vi "ACE401.vi"() -> ()   [LabVIEW 2018]
uses:
  <vilib>/registry/registry.llb/Registry RtKey.ctl
  <vilib>/registry/registry.llb/Registry SAM.ctl
  <vilib>/Utility/miscctls.llb/LVRowAndColumnUnsignedTypeDef.ctl
  <vilib>/Utility/cursorutil.llb/Set Cursor (Icon Pict).vi
  <vilib>/registry/registry.llb/Read Registry Value Simple STR.vi
panel:
  in  "Firebase URL":string
  in  "Enable IoT":bool
  out "Exp":string
  out "current time":timestamp format="%<%d/%m/%Y - %I:%M:%S %p>T"
  in  "Radio Buttons":T1(radio)
  out "Flag":bool
  in  "Action":bool
  in  "Stop Flag":bool
  out "Tank":dbl(slide) scale=0.0..100.0 scale format="%#.1g"
  in  "OP_1 2":dbl=50.0 caption="SP %" format="%3.1f"
  in  "SP_1":dbl=50.0 caption="SP %" format="%3.1f"
  in  "PV_1":dbl caption="PV %" format="%3.1f"
  out "Boolean 3":bool
  out "Multi-Segment Pipe 5":bool(c317)
  out "Multi-Segment Pipe 4":bool(c317)
  out "Multi-Segment Pipe 3":bool(c317)
  out "Multi-Segment Pipe 2":bool(c317)
  out "Boolean":bool
  out "Tank 2":dbl(slide)=58.333333333333336 scale=0.0..100.0
  out "Multi-Segment Pipe":bool(c317)
  out "Boolean 2":bool
  out "Enum":T2(ring)
  in  "Experiment Selection":u16(ring)=5 items=["On / Off Control", "P Mode", "PI Mode", "PD Mode", "PID Mode"]
  in  "Tab Control 3":enum32{"Plot2"}(tab)
  out "Waveform Chart":T3(graph)={"Register Value"=20.0, "Value"=0.0, "Register Value"=0.0}
  in  "Run":bool caption="Blank Button"
  out "Log":bool
  in  "Log Button":bool caption="Blank Button"
  in  "Constant PV":bool
  in  "Constant Outflow":bool
  in  "Anti Reset Windup":bool=TRUE
  in  "Bumpless Transfer":bool=TRUE
  in  "Pause":bool caption="Blank Button"
  in  "Single Step":bool caption="Blank Button"
  in  "Stop":bool caption="Blank Button"
  in  "Save Log":bool caption="Blank Button"
  in  "Clear":bool caption="Blank Button"
  in  "Export":bool caption="Blank Button"
  in  "help":bool caption="Blank Button"
  in  "Home":bool caption="Blank Button"
  in  "Tab Control 2":T4(tab)
  in  "Steady State Flow \n@50% of PV(LPH)":dbl(slide)=40.0 min=0.0 step=1.0 scale=0.0..100.0
  in  "Time Lag (s)":u32(slide)=1 min=1 max=10 step=1 scale=0.0..10.0
  in  "Max. Inflow (LPH)":dbl(slide)=100.0 min=0.0 step=1.0 scale=0.0..400.0
  in  "Tank Height  (cms)":dbl(slide)=25.0 min=10.0 step=1.0 scale=0.0..200.0
  in  "Tank Diameter  (cms)":dbl(slide)=10.0 min=5.0 step=1.0 scale=0.0..40.0
  in  "A / M":bool
  in  "Set Point (%)":dbl(slide)=50.0 min=0.0 max=100.0 step=0.1 scale=0.0..100.0
  in  "Process Variable (%)":dbl(slide) min=0.0 max=100.0 step=1.0 scale=0.0..100.0
  in  "Controller Output (%)":dbl(slide)=100.0 min=0.0 max=100.0 step=0.1 scale=0.0..100.0
  in  "DT s":dbl(slide)=1.0 caption="Derivative Time (s)" min=0.0 max=100.0 step=0.1 scale=0.0..20.0
  in  "IT s":dbl(slide)=30.0 caption="Integral Time (s)" min=0.0 max=100.0 step=0.1 scale=0.0..1000.0
  in  "PB %":dbl(slide)=20.0 caption="Proportional Band (%)" min=0.0 max=100.0 step=0.1 scale=0.0..400.0
  in  "Bias (%)":dbl(slide)=40.0 min=0.0 max=100.0 step=0.1 scale=0.0..100.0
  in  "Hystresis (%)":dbl(slide)=2.0 min=0.0 max=100.0 step=0.1 scale=0.0..20.0
  in  "Out Flow (%)":dbl(slide)=40.0 min=0.0 max=100.0 step=0.1 scale=0.0..100.0
  in  "Add Load":bool
  in  "PB Contribution (%)":dbl=60.0 min=0.0 max=100.0 step=0.1 format="%#.1f"
  in  "IOP":dbl=1.0 caption="IT Contribution (%)" min=0.0 max=100.0 step=0.1 format="%#.2f"
  in  "DOP":dbl=1.0 caption="DT Contribution (%)" min=0.0 max=100.0 step=0.1 format="%#.2f"
  in  "Load":dbl(slide)=10.0 caption="Load (%)" min=-50.0 max=50.0 step=1.0 scale=-100.0..100.0
  out "Table":string[][](table)
  out "out1":dbl=2.0
  in  "Array":dbl[](array[numeric])=[0.0, 0.0, 0.0, 0.0, 0.0, 0.0, 0.0, 0.0, 0.0, 0.0]
  out "err":dbl
  out "dh":dbl=2.0
  out "K":dbl
  out "Area":dbl
  out "qi":dbl=100.0
  out "i2":dbl
  out "Log Count":dbl
  out "PV % 2":dbl caption="PV %" format="%#.1f"
  out "SP % 2":dbl caption="SP %" format="%#.1f"
  # "Advanced Control Equipments\n(Ahead Traditional Control)"
  # "Two Position & PID Simulator (ACE 401)"
  # "Study Parameters"
  # "I / P Converter"
  # "Level Controller"
  # "Rotameter"
  # "Process Tank"
  # "Control Valve"
  # "Manual\nDrain Valve"
  # "Level Transmitter"
  # "Supply Tank"
  # "Pump"
  # "Select Experiment"
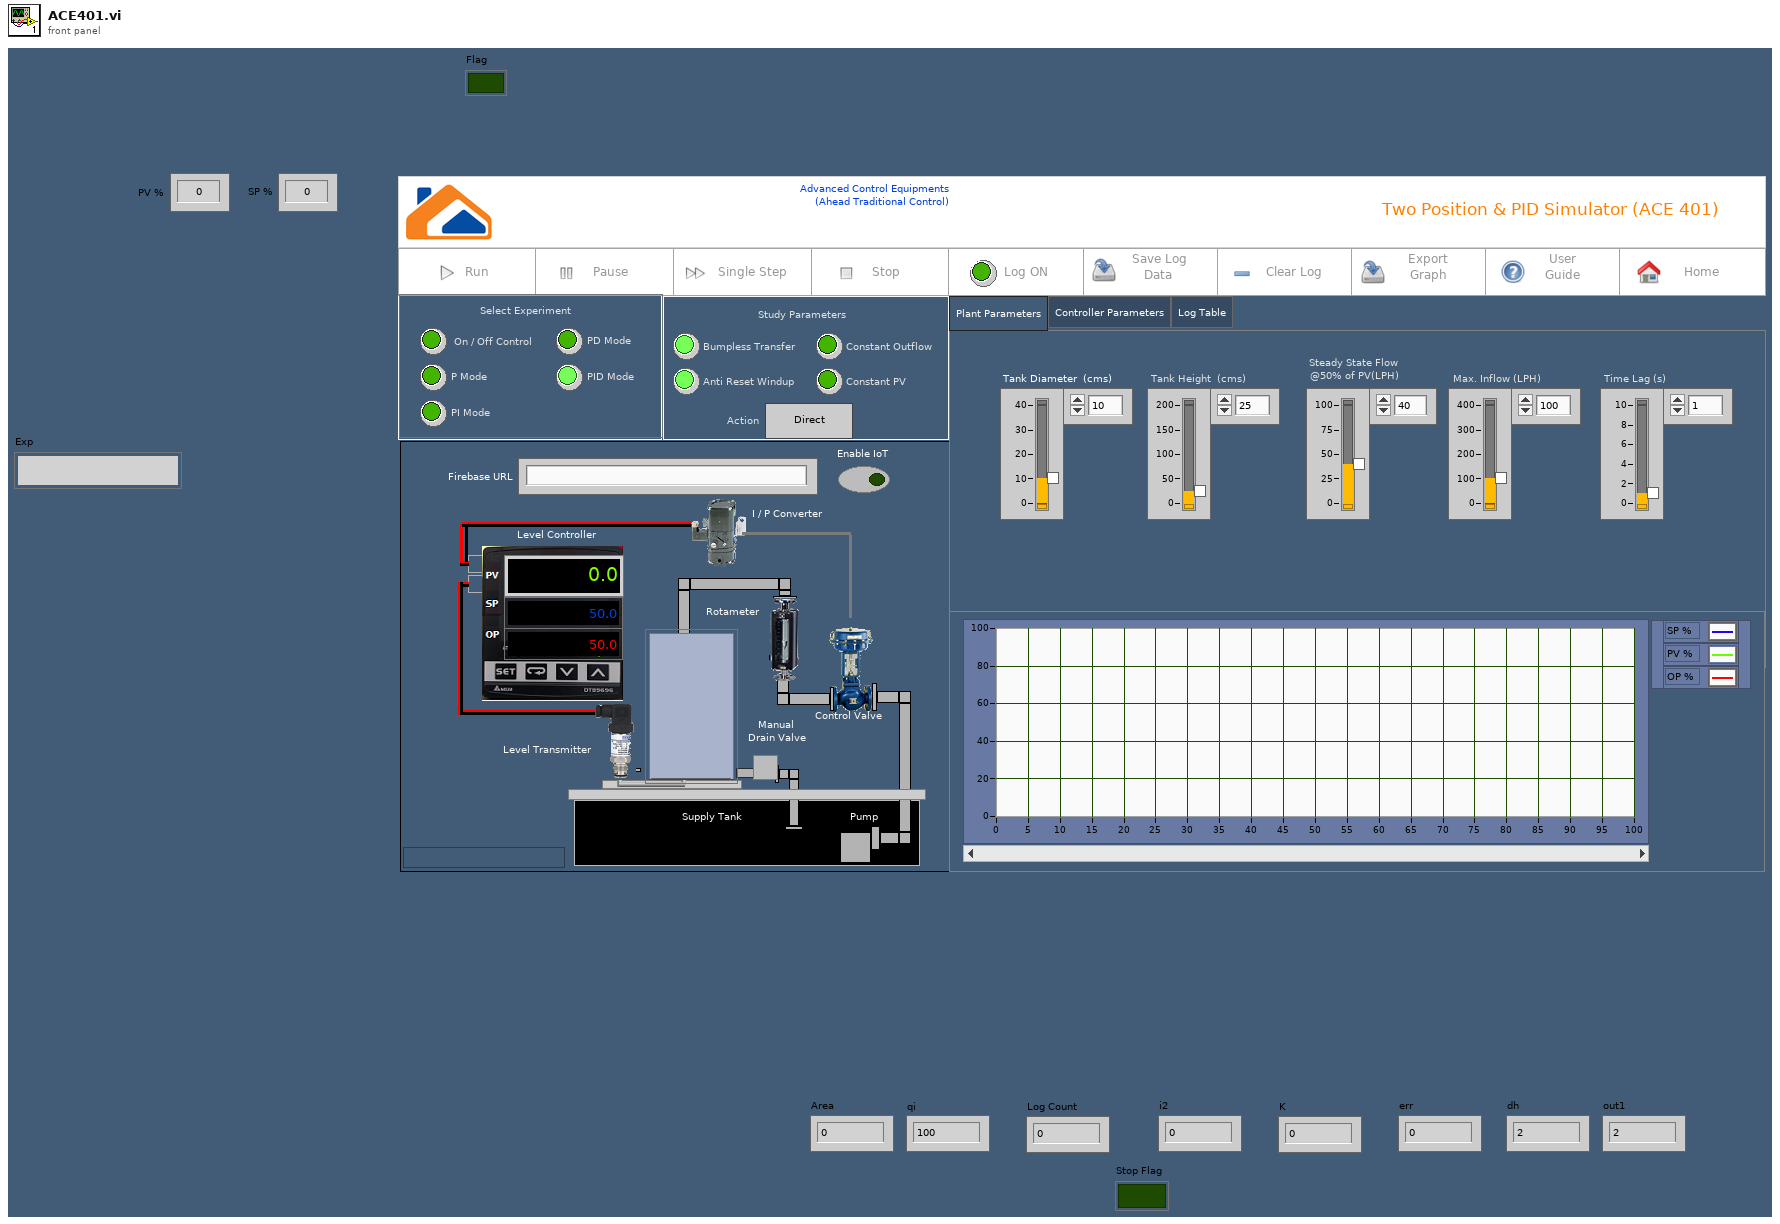
[diagram p1: front panel]
types:
  T1 = enum32{"PID Mode", "On / Off Control", "P Mode", "PI Mode", "PD Mode"}
  T2 = enum16{"Initialize", "Select Exp", "Play", "Stop", "Error", "Pause", "MainPage", "Wait"}
  T3 = cluster{"Register Value":dbl, "Value":dbl, "Register Value":dbl}
  T4 = enum32{"Plant Parameters", "Controller Parameters", "Log Table"}
  T5 = enum16{"Initialize", "Select Exp", "Play", "Stop", "Error", "Pause", "MainPage"}
  T6 = enum32{"Page Enabled", "Page Disabled", "Page Disabled & Grayed"}
  T7 = cluster{"Register Value":dbl, "Value":dbl, "Register Value":dbl}[]
  T8 = typedef "LVRowAndColumnUnsignedTypeDef.ctl" = cluster{"Row":u32, "Column":u32}
  T9 = enum8{"Enabled", "Disabled", "Disabled and Grayed Out"}
  T10 = cluster{"Set Point (%)":dbl, "pv1":dbl, "upper limit":dbl}
  T11 = typedef "Registry SAM.ctl" = enum32{"KEY_QUERY_VALUE", "KEY_SET_VALUE", "KEY_CREATE_SUB_KEY", "KEY_ENUMERATE_SUB_KEYS", "KEY_NOTIFY", "KEY_CREATE_LINK", "KEY_READ", "KEY_WRITE", "KEY_ALL_ACCESS", "KEY_READ | KEY_WRITE"}
  T12 = typedef "Registry RtKey.ctl" = enum32{"HKEY_CLASSES_ROOT", "HKEY_CURRENT_USER", "HKEY_LOCAL_MACHINE", "HKEY_USERS", "HKEY_PERFORMANCE_DATA", "HKEY_CURRENT_CONFIG", "HKEY_DYN_DATA"}
  T13 = typedef "imagedata.ctl" = cluster{"image type":i32, "image depth":i32, "image":u8[], "mask":u8[], "colors":u32[], "Rectangle":cluster{"left":i16, "top":i16, "right":i16, "bottom":i16}}
  T14 = typedef "Registry refnum.ctl" = refnum<k1>
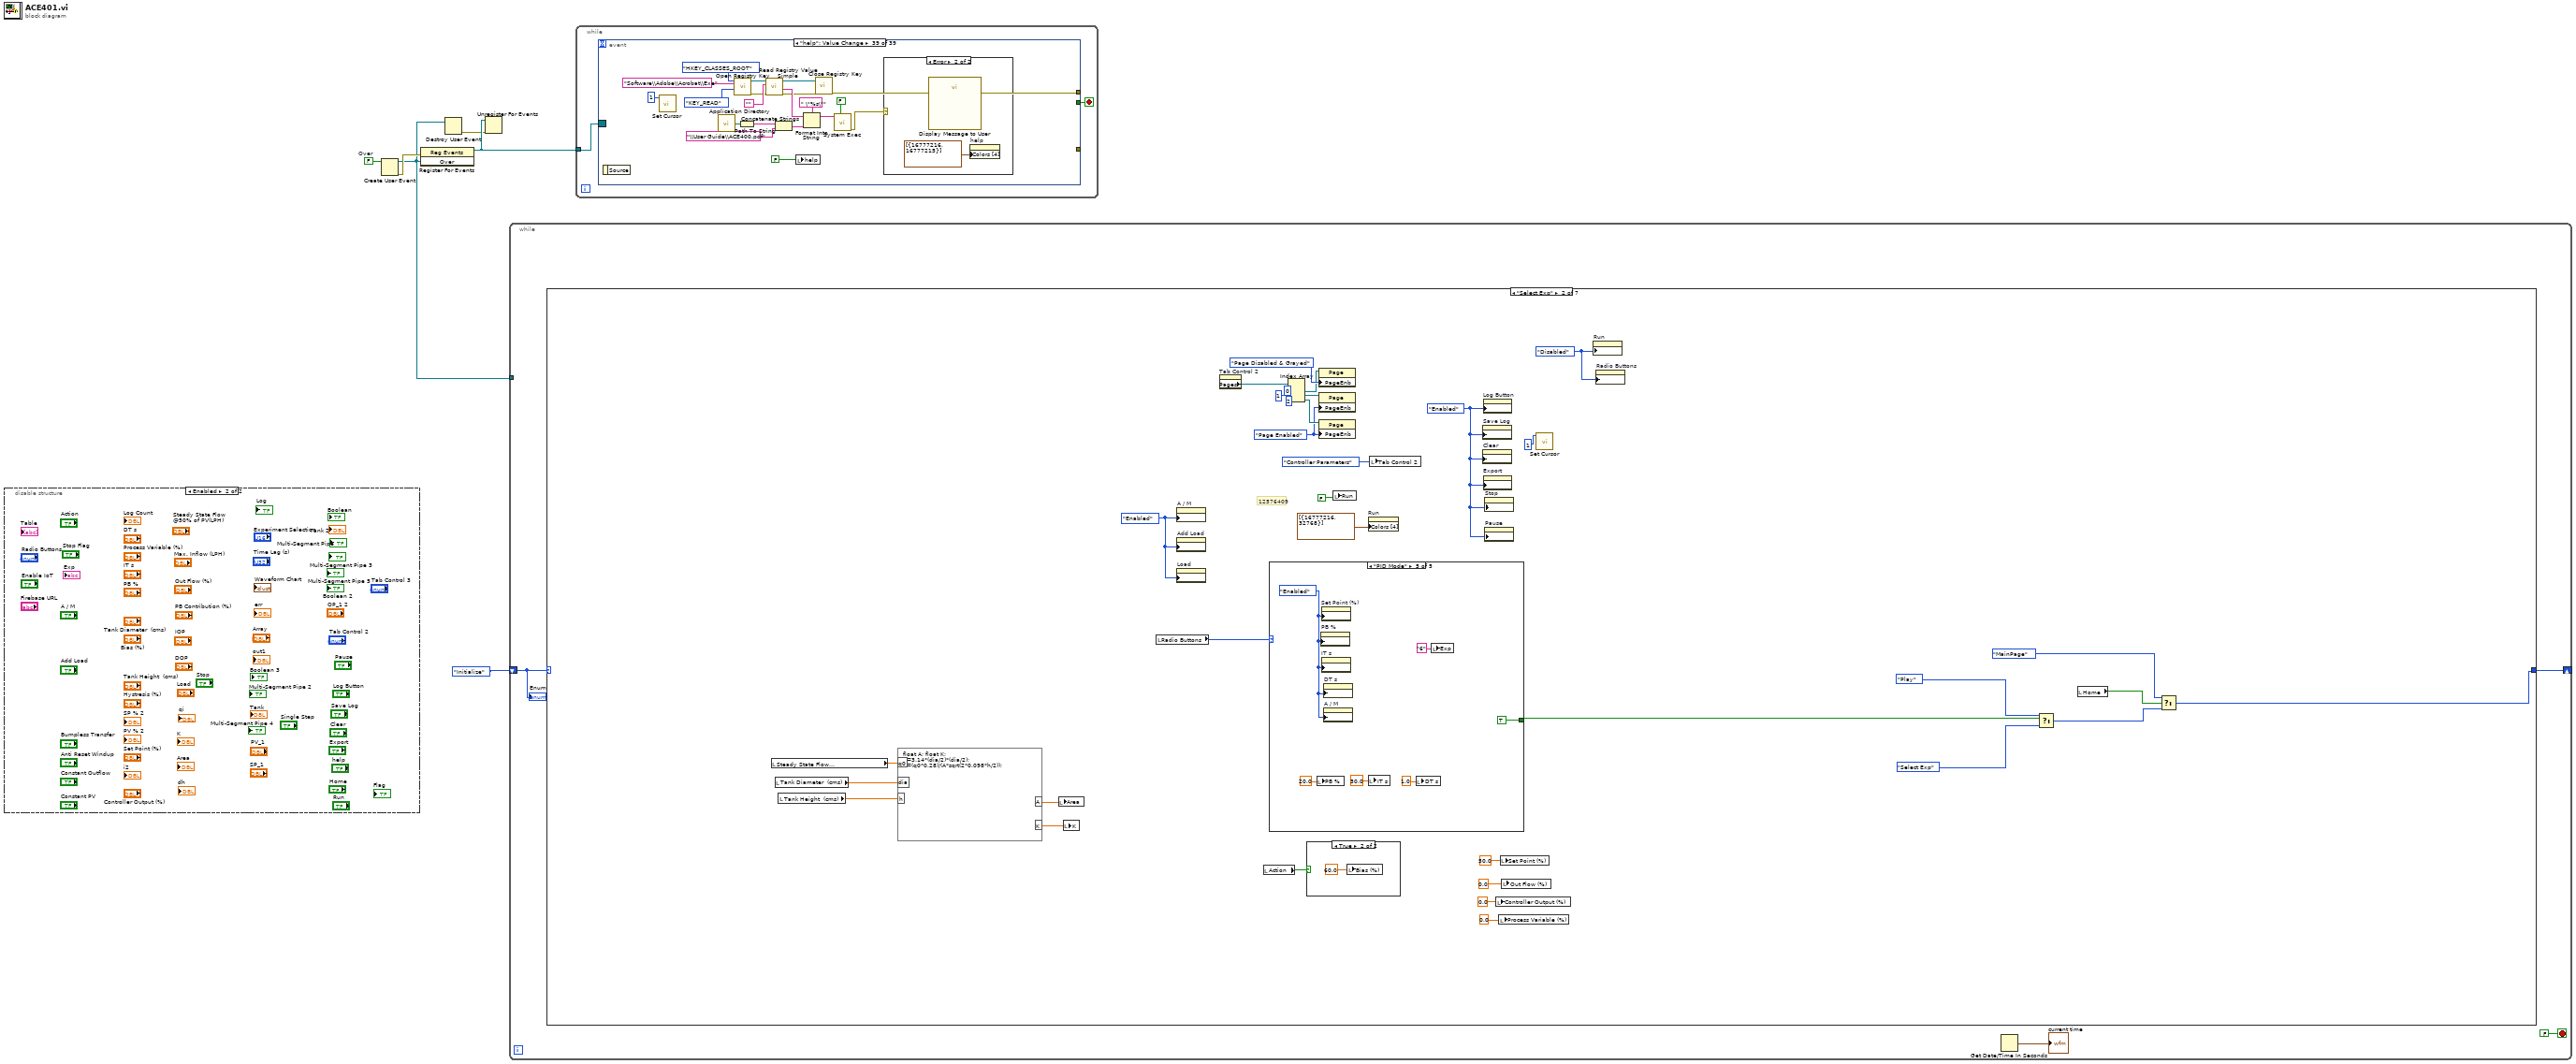
[diagram p0: block diagram]
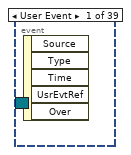
[diagram p2: hidden frame]
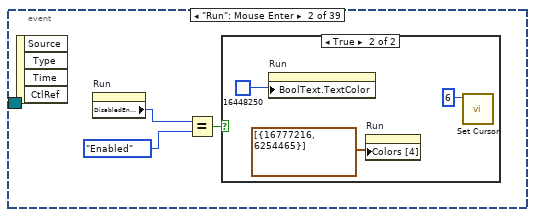
[diagram p3: hidden frame]
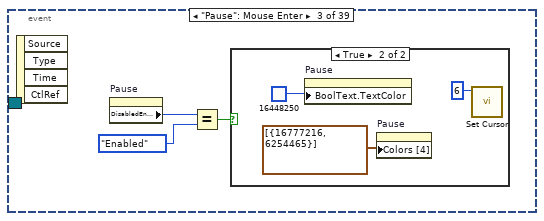
[diagram p5: hidden frame]
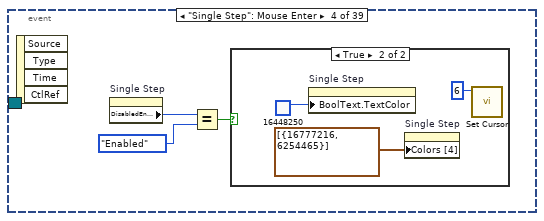
[diagram p7: hidden frame]
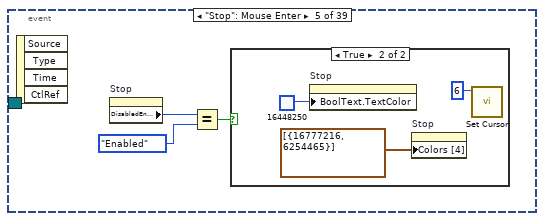
[diagram p9: hidden frame]
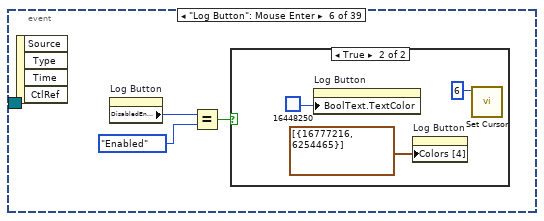
[diagram p11: hidden frame]
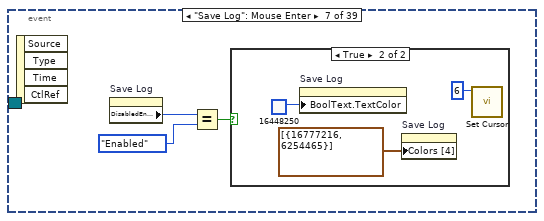
[diagram p13: hidden frame]
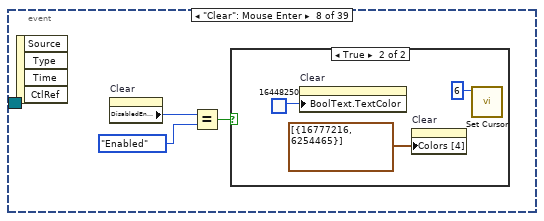
[diagram p15: hidden frame]
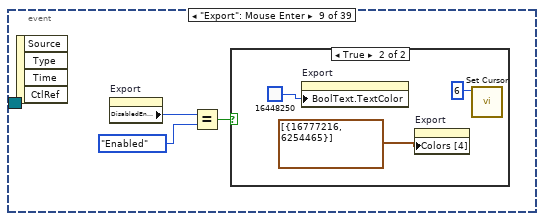
[diagram p17: hidden frame]
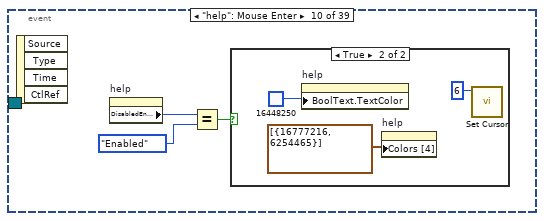
[diagram p19: hidden frame]
diagram:
  w4 = FALSE  # Over
  n1 = disable-structure shown="Enabled" {
    frame Disabled {
    }
    frame Enabled {
    }
  }
  n2 = Create User Event(user event datatype=w4) -> (user event=w2:refnum<user-event>, error out=w5:errorcluster)  [unwired: 1 in]
  n3 = register-events(error in=w5, w2) -> (reference out=w3:refnum<event-registration>)  [unwired: 1 in, 1 out]
  n4 = Unregister For Events(event registration refnum=w3) -> (error out=w1:errorcluster)  [unwired: 1 in]
  n5 = Destroy User Event(user event=w2, error in=w1) -> ()  [unwired: 1 out]
  n6 = while {
    shift-right: [w10] -> _
    shift-left: T2."Initialize" -> [w8]
    tunnel: w2 -> [_]
    stop <- FALSE stop-if-true
    n7 = case shown="\"Select Exp\"" w8 {
      tunnel: [w17 w75 w125 w682 w692 w698 _] -> w10
      frame "Initialize", Default {
        n8 = flat-sequence {
          frame #0 {
            w19 = T9."Disabled and Grayed Out" ("Disabled")
            w18 = T9."Enabled" ("Disabled")
            w22 = FALSE ("Stop Button")
            w31 = T6."Page Disabled & Grayed" ("Page Enabled State")
            w20 = T9."Disabled" ("Disabled")
            w21 = FALSE ("Log Button")
            w37 = 0.0 ("Log Count")
            n9 = local read "Action"() -> (w23:bool)
            n10 = property on="A / M" class="Bool (strict)"("BoolText.Text"="Auto" ("Boolean Text.Text")) -> ()  [unwired: 2 in, 2 out]
            n11 = case shown="False" w23 {
              frame True {
                n12 = property on="Array" class="Arr (strict)"("Value"=dbl[] [100.0, 100.0, 100.0, 100.0, 100.0, 100.0, 100.0, 100.0, 100.0, 100.0] ("Array")) -> ()  [unwired: 2 in, 2 out]
              }
              frame False {
                n13 = property on="Array" class="Arr (strict)"("Value"=dbl[] [0.0, 0.0, 0.0, 0.0, 0.0, 0.0, 0.0, 0.0, 0.0, 0.0] ("Array")) -> ()  [unwired: 2 in, 2 out]
              }
            }
            n14 = invoke on="Table" class="Tbl (strict)" method="Reinit To Default"() -> ()  [unwired: 3 in, 3 out]
            n15 = property on="Table" class="Tbl (strict)"("Value"=string[][] [] ("Table")) -> ()  [unwired: 2 in, 2 out]
            n16 = local write "Log Button"(w21) -> ()
            n17 = local write "Single Step"(w21) -> ()
            n18 = local write "Stop Flag"(w21) -> ()
            n19 = local write "A / M"(w21) -> ()
            n20 = local write "Pause"(w21) -> ()
            n21 = local write "Clear"(w21) -> ()
            n22 = local write "Stop"(w21) -> ()
            n23 = property on="Waveform Chart" class="WFChart (strict)"("History Data"=T7 []) -> ()  [unwired: 2 in, 2 out]
            n24 = local write "Single Step"(w22) -> ()
            n25 = local write "Pause"(w22) -> ()
            n26 = local write "Stop"(w22) -> ()
            n27 = local write "Process Variable (%)"(w37) -> ()
            n28 = local write "PB Contribution (%)"(w37) -> ()
            n29 = property on="Tab Control 2" class="TabCtl (strict)"() -> ("Pages"=w28:refnum<vi>[])  [unwired: 2 in, 2 out]
            n30 = local write "Log Count"(w37) -> ()
            n31 = local write "Bias (%)"(w37) -> ()
            n32 = local write "OP_1 2"(w37) -> ()
            n33 = local write "i2"(w37) -> ()
            n34 = local write "DOP"(w37) -> ()
            n35 = local write "PV_1"(w37) -> ()
            n36 = local write "IOP"(w37) -> ()
            n37 = local write "dh"(w37) -> ()
            n38 = Index Array(array=w28, index #1=0 ("index"), index #2=1 ("index"), index #3=2 ("index")) -> (element #1=w25:refnum<vi>, element #2=w30:refnum<vi>, element #3=w32:refnum<vi>)
            n39 = local write "qi"(100.0 ("qi")) -> ()
            n40 = local write "Tab Control 2"(T4."Plant Parameters" ("Tab Control 2")) -> ()
            n41 = local write "SP_1"(50.0 ("qi")) -> ()
            n42 = property on="Table" class="Tbl (strict)"("Index Values"=T8 {"Row"=0, "Column"=0}) -> ()  [unwired: 2 in, 2 out]
            n43 = property on="Log" class="Bool (strict)"("Blinking"=FALSE) -> ()  [unwired: 2 in, 2 out]
            n44 = property class="Page"(reference=w25, "PageEnb"=T6."Page Enabled" ("Page Enabled State")) -> ()  [unwired: 1 in, 2 out]
            n45 = property class="Page"(reference=w30, "PageEnb"=w31) -> ()  [unwired: 1 in, 2 out]
            n46 = property class="Page"(reference=w32, "PageEnb"=w31) -> ()  [unwired: 1 in, 2 out]
            n47 = property on="Log Button" class="Bool (strict)"("DisabledEnum"=w20) -> ()  [unwired: 2 in, 2 out]
            n48 = property on="Save Log" class="Bool (strict)"("DisabledEnum"=w20) -> ()  [unwired: 2 in, 2 out]
            n49 = property on="Clear" class="Bool (strict)"("DisabledEnum"=w20) -> ()  [unwired: 2 in, 2 out]
            n50 = property on="Export" class="Bool (strict)"("DisabledEnum"=w20) -> ()  [unwired: 2 in, 2 out]
            n51 = property on="Stop" class="Bool (strict)"("DisabledEnum"=w20) -> ()  [unwired: 2 in, 2 out]
            n52 = property on="Single Step" class="Bool (strict)"("DisabledEnum"=w20) -> ()  [unwired: 2 in, 2 out]
            n53 = property on="Pause" class="Bool (strict)"("DisabledEnum"=w20) -> ()  [unwired: 2 in, 2 out]
            n54 = property on="Log" class="Bool (strict)"("DisabledEnum"=w20) -> ()  [unwired: 2 in, 2 out]
            n55 = property on="Run" class="Bool (strict)"("DisabledEnum"=w18) -> ()  [unwired: 2 in, 2 out]
            n56 = property on="Radio Buttons" class="RadioBtnsControl (strict)"("DisabledEnum"=w18) -> ()  [unwired: 2 in, 2 out]
            n57 = property on="Home" class="Bool (strict)"("DisabledEnum"=w18) -> ()  [unwired: 2 in, 2 out]
            n58 = property on="help" class="Bool (strict)"("DisabledEnum"=w18) -> ()  [unwired: 2 in, 2 out]
            n59 = property on="Action" class="Bool (strict)"("DisabledEnum"=w18) -> ()  [unwired: 2 in, 2 out]
            n60 = property on="Out Flow (%)" class="Slide (strict)"("DisabledEnum"=w19) -> ()  [unwired: 2 in, 2 out]
            n61 = property on="PB %" class="Slide (strict)"("DisabledEnum"=w19) -> ()  [unwired: 2 in, 2 out]
            n62 = property on="IT s" class="Slide (strict)"("DisabledEnum"=w19) -> ()  [unwired: 2 in, 2 out]
            n63 = property on="DT s" class="Slide (strict)"("DisabledEnum"=w19) -> ()  [unwired: 2 in, 2 out]
            n64 = property on="Process Variable (%)" class="Slide (strict)"("DisabledEnum"=w19) -> ()  [unwired: 2 in, 2 out]
            n65 = property on="Controller Output (%)" class="Slide (strict)"("DisabledEnum"=w19) -> ()  [unwired: 2 in, 2 out]
            n66 = property on="Bias (%)" class="Slide (strict)"("DisabledEnum"=w19) -> ()  [unwired: 2 in, 2 out]
            n67 = property on="Hystresis (%)" class="Slide (strict)"("DisabledEnum"=w19) -> ()  [unwired: 2 in, 2 out]
          }
        }
        n68 = local read "Run"() -> (w11:bool)
        n69 = local read "Home"() -> (w12:bool)
        n70 = Select(t=T5."Select Exp", s=w11, f=T5."Initialize") -> (s? t:f=w16:T5)
        n71 = Select(t=T5."MainPage", s=w12, f=w16) -> (s? t:f=w17:T5)
      }
      frame "Select Exp" {
        w47 = T9."Enabled" ("Disabled")
        w48 = T9."Disabled" ("Disabled")
        w55 = T6."Page Enabled" ("Page Enabled State")
        w61 = T9."Enabled" ("Disabled")
        # "12576409"
        n72 = local read "Steady State Flow \n@50% of PV(LPH)"() -> (w69:dbl)
        n73 = local read "Tank Diameter  (cms)"() -> (w68:dbl)
        n74 = local read "Tank Height  (cms)"() -> (w67:dbl)
        n75 = formula code="float A; float K; \nA=3.14*(dia/2)*(dia/2);\nK=(q0*0.28)/(A*sqrt(2*0.098*h/2));"("q0"=w69, "dia"=w68, "h"=w67) -> ("A"=w70:dbl, "K"=w71:dbl)
        n76 = local write "Area"(w70) -> ()
        n77 = local write "K"(w71) -> ()
        n78 = local read "Radio Buttons"() -> (w44:T1)
        n79 = property on="A / M" class="Bool (strict)"("DisabledEnum"=w61) -> ()  [unwired: 2 in, 2 out]
        n80 = property on="Add Load" class="Bool (strict)"("DisabledEnum"=w61) -> ()  [unwired: 2 in, 2 out]
        n81 = property on="Load" class="Slide (strict)"("DisabledEnum"=w61) -> ()  [unwired: 2 in, 2 out]
        n82 = property on="Tab Control 2" class="TabCtl (strict)"() -> ("Pages"=w52:refnum<vi>[])  [unwired: 2 in, 2 out]
        n83 = local read "Action"() -> (w66:bool)
        n84 = case shown="\"PID Mode\"" w44 {
          tunnel: [TRUE ("wait until completion? (T)") TRUE ("wait until completion? (T)") TRUE ("wait until completion? (T)") TRUE ("wait until completion? (T)") TRUE ("wait until completion? (T)")] -> w45
          frame "On / Off Control", Default {
            w83 = T9."Enabled" ("Disabled")
            # "On/Off"
            n85 = local read "Action"() -> (w82:bool)
            n86 = local write "PB %"(0.0 ("PB %")) -> ()
            n87 = property on="Hystresis (%)" class="Slide (strict)"("DisabledEnum"=w83) -> ()  [unwired: 2 in, 2 out]
            n88 = property on="Set Point (%)" class="Slide (strict)"("DisabledEnum"=w83) -> ()  [unwired: 2 in, 2 out]
            n89 = local write "IT s"(0.0 ("IT s")) -> ()
            n90 = case shown="True" w82 {
              frame False {
                n91 = local write "Controller Output (%)"(100.0 ("PB %")) -> ()
              }
              frame True {
                n92 = local write "Controller Output (%)"(0.0 ("PB %")) -> ()
              }
            }
            n93 = local write "DT s"(0.0 ("DT s")) -> ()
            n94 = local write "Exp"("2" ("Exp")) -> ()
          }
          frame "P Mode" {
            w94 = T9."Enabled" ("Disabled")
            n95 = local write "PB %"(20.0 ("PB %")) -> ()
            n96 = property on="PB %" class="Slide (strict)"("DisabledEnum"=w94) -> ()  [unwired: 2 in, 2 out]
            n97 = property on="Set Point (%)" class="Slide (strict)"("DisabledEnum"=w94) -> ()  [unwired: 2 in, 2 out]
            n98 = property on="Bias (%)" class="Slide (strict)"("DisabledEnum"=w94) -> ()  [unwired: 2 in, 2 out]
            n99 = property on="A / M" class="Bool (strict)"("DisabledEnum"=w94) -> ()  [unwired: 2 in, 2 out]
            n100 = local write "IT s"(0.0 ("IT s")) -> ()
            n101 = local write "DT s"(0.0 ("DT s")) -> ()
            n102 = local write "Exp"("3" ("Exp")) -> ()
          }
          frame "PI Mode" {
            w100 = T9."Enabled" ("Disabled")
            n103 = local write "PB %"(20.0 ("PB %")) -> ()
            n104 = property on="PB %" class="Slide (strict)"("DisabledEnum"=w100) -> ()  [unwired: 2 in, 2 out]
            n105 = property on="Set Point (%)" class="Slide (strict)"("DisabledEnum"=w100) -> ()  [unwired: 2 in, 2 out]
            n106 = property on="IT s" class="Slide (strict)"("DisabledEnum"=w100) -> ()  [unwired: 2 in, 2 out]
            n107 = property on="A / M" class="Bool (strict)"("DisabledEnum"=w100) -> ()  [unwired: 2 in, 2 out]
            n108 = local write "IT s"(30.0 ("IT s")) -> ()
            n109 = local write "DT s"(0.0 ("DT s")) -> ()
            n110 = local write "Exp"("4" ("Exp")) -> ()
          }
          frame "PD Mode" {
            w106 = T9."Enabled" ("Disabled")
            n111 = local write "PB %"(20.0 ("PB %")) -> ()
            n112 = property on="PB %" class="Slide (strict)"("DisabledEnum"=w106) -> ()  [unwired: 2 in, 2 out]
            n113 = property on="Set Point (%)" class="Slide (strict)"("DisabledEnum"=w106) -> ()  [unwired: 2 in, 2 out]
            n114 = property on="DT s" class="Slide (strict)"("DisabledEnum"=w106) -> ()  [unwired: 2 in, 2 out]
            n115 = property on="A / M" class="Bool (strict)"("DisabledEnum"=w106) -> ()  [unwired: 2 in, 2 out]
            n116 = local write "IT s"(0.0 ("IT s")) -> ()
            n117 = local write "DT s"(1.0 ("DT s")) -> ()
            n118 = local write "Exp"("5" ("Exp")) -> ()
          }
          frame "PID Mode" {
            w112 = T9."Enabled" ("Disabled")
            n119 = local write "PB %"(20.0 ("PB %")) -> ()
            n120 = property on="PB %" class="Slide (strict)"("DisabledEnum"=w112) -> ()  [unwired: 2 in, 2 out]
            n121 = property on="Set Point (%)" class="Slide (strict)"("DisabledEnum"=w112) -> ()  [unwired: 2 in, 2 out]
            n122 = property on="IT s" class="Slide (strict)"("DisabledEnum"=w112) -> ()  [unwired: 2 in, 2 out]
            n123 = property on="DT s" class="Slide (strict)"("DisabledEnum"=w112) -> ()  [unwired: 2 in, 2 out]
            n124 = property on="A / M" class="Bool (strict)"("DisabledEnum"=w112) -> ()  [unwired: 2 in, 2 out]
            n125 = local write "IT s"(30.0 ("IT s")) -> ()
            n126 = local write "DT s"(1.0 ("DT s")) -> ()
            n127 = local write "Exp"("6" ("Exp")) -> ()
          }
        }
        n128 = Index Array(array=w52, index #1=0 ("index"), index #2=1 ("index"), index #3=2 ("index")) -> (element #1=w49:refnum<vi>, element #2=w54:refnum<vi>, element #3=w56:refnum<vi>)
        n129 = case shown="True" w66 {
          frame False {
            n130 = local write "Bias (%)"(40.0 ("PB %")) -> ()
          }
          frame True {
            n131 = local write "Bias (%)"(60.0 ("PB %")) -> ()
          }
        }
        n132 = property class="Page"(reference=w49, "PageEnb"=T6."Page Disabled & Grayed" ("Page Enabled State")) -> ()  [unwired: 1 in, 2 out]
        n133 = property class="Page"(reference=w54, "PageEnb"=w55) -> ()  [unwired: 1 in, 2 out]
        n134 = property class="Page"(reference=w56, "PageEnb"=w55) -> ()  [unwired: 1 in, 2 out]
        n135 = local write "Run"(FALSE ("Blinking")) -> ()
        n136 = property on="Run" class="Bool (strict)"("Colors [4]"=cluster{u32, u32}[] [{16777216, 32768}]) -> ()  [unwired: 2 in, 2 out]
        n137 = local write "Tab Control 2"(T4."Controller Parameters" ("Tab Control 2")) -> ()
        n138 = property on="Save Log" class="Bool (strict)"("DisabledEnum"=w47) -> ()  [unwired: 2 in, 2 out]
        n139 = property on="Clear" class="Bool (strict)"("DisabledEnum"=w47) -> ()  [unwired: 2 in, 2 out]
        n140 = property on="Log Button" class="Bool (strict)"("DisabledEnum"=w47) -> ()  [unwired: 2 in, 2 out]
        n141 = property on="Export" class="Bool (strict)"("DisabledEnum"=w47) -> ()  [unwired: 2 in, 2 out]
        n142 = property on="Stop" class="Bool (strict)"("DisabledEnum"=w47) -> ()  [unwired: 2 in, 2 out]
        n143 = property on="Pause" class="Bool (strict)"("DisabledEnum"=w47) -> ()  [unwired: 2 in, 2 out]
        n144 = local write "Controller Output (%)"(0.0 ("DT s")) -> ()
        n145 = local write "Process Variable (%)"(0.0 ("DT s")) -> ()
        n146 = local write "Set Point (%)"(50.0 ("PB %")) -> ()
        n147 = local write "Out Flow (%)"(0.0 ("IT s")) -> ()
        n148 = call-poly <vilib>:"Set Cursor.vi"("icon"=u16 1) -> ()  [unwired: 9 in, 2 out]
        n149 = property on="Run" class="Bool (strict)"("DisabledEnum"=w48) -> ()  [unwired: 2 in, 2 out]
        n150 = property on="Radio Buttons" class="RadioBtnsControl (strict)"("DisabledEnum"=w48) -> ()  [unwired: 2 in, 2 out]
        n151 = Select(t=T5."Play", s=w45, f=T5."Select Exp") -> (s? t:f=w76:T5)
        n152 = local read "Home"() -> (w77:bool)
        n153 = Select(t=T5."MainPage", s=w77, f=w76) -> (s? t:f=w75:T5)
      }
      frame "Play" {
        w116 = T9."Disabled and Grayed Out" ("Disabled")
        w124 = T9."Enabled" ("Disabled")
        w123 = T9."Disabled" ("Disabled")
        n154 = local read "Enable IoT"() -> (w113:bool)
        n155 = local read "Radio Buttons"() -> (w144:T1)
        n156 = case shown="True" w113 {
          frame False {
          }
          frame True {
            n157 = flat-sequence {
              tunnel: [w154] -> w146
              tunnel: [w149] -> w145
              tunnel: w146 -> [_]
              tunnel: w145 -> [w164]
              tunnel: [w163] -> _
              frame #0 {
                n158 = local read "A / M"() -> (w153:bool)
                n159 = local read "Process Variable (%)"() -> (w152:dbl)
                n160 = local read "Firebase URL"() -> (w149:string)
                n161 = local read "Exp"() -> (w151:string)
                n162 = local read "Controller Output (%)"() -> (w150:dbl)
                n163 = local read "Set Point (%)"() -> (w148:dbl)
                n164 = Wait Until Next ms Multiple(millisecond multiple=u32 100 ("milliseconds to wait")) -> ()  [unwired: 1 out]
                n165 = call "Write_Firebase_Basic.vi"("Firebase URL"=w149, "PV (%)"=w152, "Experiment"=w151, "OP (%)"=w150, "SP (%)"=w148, "Auto"=w153) -> ("error out"=w154:errorcluster)  [unwired: 9 in]
              }
              frame #1 {
                n166 = call "Read_Firebase_Basic.vi"("Firebase URL"=w164) -> ("OP Manual"=w156:dbl, "Set Point (%)"=w162:dbl, "Bias (%)"=w157:dbl, "Hystresis (%)"=w158:dbl, "AM"=w155:bool, "PB %"=w159:dbl, "IT s"=w160:dbl, "DT s"=w161:dbl, "error out"=w163:errorcluster)  [unwired: 1 in]
                n167 = case shown="True" w155 {
                  tunnel: w156 -> [_ w165]
                  frame False {
                  }
                  frame True {
                    n168 = local write "Controller Output (%)"(w165) -> ()
                  }
                }
                n169 = local write "Hystresis (%)"(w158) -> ()
                n170 = local write "Set Point (%)"(w162) -> ()
                n171 = local write "A / M"(w155) -> ()
                n172 = local write "Bias (%)"(w157) -> ()
                n173 = local write "PB %"(w159) -> ()
                n174 = local write "DT s"(w161) -> ()
                n175 = local write "IT s"(w160) -> ()
              }
            }
          }
        }
        n176 = local read "Anti Reset Windup"() -> (w129:bool)
        n177 = local read "Process Variable (%)"() -> (w130:dbl)
        n178 = local read "Set Point (%)"() -> (w138:dbl)
        n179 = local read "Bumpless Transfer"() -> (w136:bool)
        n180 = local read "Bias (%)"() -> (w134:dbl)
        n181 = local read "Constant PV"() -> (w133:bool)
        n182 = local read "PB %"() -> (w141:dbl)
        n183 = local read "IT s"() -> (w142:dbl)
        n184 = local read "DT s"() -> (w143:dbl)
        n185 = local read "err"() -> (w137:dbl)
        n186 = local read "Controller Output (%)"() -> (w140:dbl)
        n187 = local read "A / M"() -> (w132:bool)
        n188 = Boolean To (0,1)(Boolean=w129) -> (0, 1=w128:i16)
        n189 = Boolean To (0,1)(Boolean=w136) -> (0, 1=w135:i16)
        n190 = Boolean To (0,1)(Boolean=w133) -> (0, 1=w127:i16)
        n191 = Boolean To (0,1)(Boolean=w132) -> (0, 1=w131:i16)
        n192 = case shown="\"PID Mode\", Default" w144 {
          tunnel: w143 -> [w232 w318 w409 w503 w596]
          tunnel: w142 -> [w233 w319 w410 w504 w597]
          tunnel: w141 -> [w235 w321 w412 w506 w599]
          tunnel: w140 -> [w237 w323 w414 w508 w601]
          tunnel: w138 -> [w236 w322 w413 w507 w600]
          tunnel: w131 -> [w234 w320 w411 w505 w598]
          tunnel: w137 -> [w230 w316 w407 w501 w594]
          tunnel: w135 -> [w225 w311 w401 w496 w588]
          tunnel: w134 -> [w226 w312 w402 w497 w589]
          tunnel: w127 -> [w224 w310 w400 w495 w587]
          tunnel: w130 -> [w223 w309 w399 w494 w586]
          tunnel: w128 -> [w221 w307 w397 w492 w584]
          tunnel: [w217 w303 w393 w488 w580] -> w115
          frame "On / Off Control" {
            # "On/Off Mode"
            n193 = flat-sequence {
              tunnel: [w259] -> w239
              tunnel: [w246] -> w238
              tunnel: w239 -> [w287]
              tunnel: w238 -> [w288]
              tunnel: w237 -> [w286]
              tunnel: w236 -> [w285]
              tunnel: w235 -> [_]
              tunnel: w234 -> [w284]
              tunnel: w233 -> [_]
              tunnel: w232 -> [_]
              tunnel: [w283] -> w231
              tunnel: w230 -> [_]
              tunnel: [w282] -> w229
              tunnel: [w281] -> w228
              tunnel: [w280] -> w227
              tunnel: w226 -> [_]
              tunnel: w225 -> [_]
              tunnel: w224 -> [w279]
              tunnel: w223 -> [w278]
              tunnel: [w277] -> w222
              tunnel: w221 -> [_]
              tunnel: [w270] -> w220
              tunnel: [w269] -> w219
              tunnel: [w268] -> w218
              tunnel: w236 -> [w302]
              tunnel: w231 -> [w300]
              tunnel: w229 -> [w299]
              tunnel: w228 -> [w298]
              tunnel: w227 -> [w297]
              tunnel: w222 -> [w296]
              tunnel: w220 -> [w295]
              tunnel: w219 -> [w291]
              tunnel: w218 -> [w292]
              tunnel: [w289] -> w217
              frame #0 {
                n194 = local read "Process Variable (%)"() -> (w260:dbl)
                n195 = local read "Out Flow (%)"() -> (w263:dbl)
                n196 = local read "Constant Outflow"() -> (w245:bool)
                n197 = local read "Action"() -> (w264:bool)
                n198 = local read "Add Load"() -> (w242:bool)
                n199 = local read "Load"() -> (w241:dbl)
                n200 = local read "qi"() -> (w262:dbl)
                n201 = local read "out1"() -> (w261:dbl)
                n202 = local read "Tank Height  (cms)"() -> (w253:dbl)
                n203 = local read "Max. Inflow (LPH)"() -> (w254:dbl)
                n204 = local read "Area"() -> (w256:dbl)
                n205 = local read "K"() -> (w255:dbl)
                n206 = Boolean To (0,1)(Boolean=w264) -> (0, 1=w246:i16)
                n207 = Boolean To (0,1)(Boolean=w242) -> (0, 1=w240:i16)
                n208 = Boolean To (0,1)(Boolean=w245) -> (0, 1=w244:i16)
                n209 = case shown="0, Default" w244 {
                  frame 1 {
                    n210 = property on="Out Flow (%)" class="Slide (strict)"("DisabledEnum"=T9."Enabled" ("Disabled")) -> ()  [unwired: 2 in, 2 out]
                  }
                  frame 0, Default {
                    n211 = property on="Out Flow (%)" class="Slide (strict)"("DisabledEnum"=T9."Disabled and Grayed Out" ("Disabled")) -> ()  [unwired: 2 in, 2 out]
                  }
                }
                n212 = formula code="float dh; float pv; float pv_cm;\n\ndh=(qi-q0)*0.28/A;\npv=(100/h)*dh; \npv1=pv+pv1;\npv_cm=pv1/4;    \n\nif (flow==0) {\nq0=K*A*(sqrt(2*0.098*pv_cm)/0.28);\n}\n\nif (act==0){\nqi=qimax-(out*qimax/100);}\nelse{\nqi=out*qimax/100;    \n}\n\nif (add==1){\npv1=pv1+load;}"("qi"=w262, "act"=w246, "q0"=w263, "out"=w261, "pv1"=w260, "A"=w256, "K"=w255, "qimax"=w254, "h"=w253, "flow"=w244, "add"=w240, "load"=w241) -> ("pv1"=w243:dbl, "qi"=w252:dbl, "q0"=w249:dbl, "dh"=w247:dbl)
                n213 = local write "dh"(w247) -> ()
                n214 = local write "qi"(w252) -> ()
                n215 = In Range and Coerce(upper limit=100.0, x=w249, lower limit=0.0) -> (coerced(x)=w248:dbl)  [unwired: 1 out]
                n216 = local write "Out Flow (%)"(w248) -> ()
                n217 = In Range and Coerce(upper limit=100.0, x=w243, lower limit=0.0) -> (coerced(x)=w259:dbl)  [unwired: 1 out]
              }
              frame #1 {
                n218 = local read "Hystresis (%)"() -> (w267:dbl)
                n219 = formula code="if (act==0)\n{\nif (pv1 >= sp1+(hys*0.5))\nout=100;\n else if (pv1 <= sp1-(hys*0.5))\n  out=0;\n}\nelse\n{\nif (pv1 >= sp1+(hys*0.5))\nout=0;\n else if (pv1 <= sp1-(hys*0.5))\n  out=100;\n}\nif (AM==1)\n{\nout=OP;\n}\n\nif (PV==1){\npv1=PV1;\n}"("sp1"=w285, "pv1"=w287, "act"=w288, "AM"=w284, "OP"=w286, "hys"=w267, "PV"=w279, "PV1"=w278) -> ("out"=w268:dbl, "error"=w283:dbl, "iop"=w281:dbl, "dop"=w282:dbl, "pop"=w280:dbl, "pv1"=w277:dbl)
                n220 = property on="Array" class="Arr (strict)"() -> ("Value"=w271:dbl[])  [unwired: 2 in, 2 out]
                n221 = local read "Time Lag (s)"() -> (w272:u32)
                n222 = Rotate 1D Array(1:w271, 2:1 ("n")) -> (0:w274:dbl[])
                n223 = Decrement(x=w272) -> (x-1=w273:u32)
                n224 = Replace Array Subset(array=w274, new element=w268, index=0) -> (w270:dbl[])
                n225 = Index Array(array=w270, index=w273) -> (element=w269:dbl)
              }
              frame #2 {
                n226 = local write "out1"(w291) -> ()
                n227 = property on="Array" class="Arr (strict)"("Value"=w295) -> ()  [unwired: 2 in, 2 out]
                n228 = In Range and Coerce(upper limit=100.0, x=w292, lower limit=0.0) -> (coerced(x)=w289:dbl)  [unwired: 1 out]
                n229 = Bundle("Set Point (%)"=w302, "pv1"=w296, "upper limit"=w289) -> (w301:T10)  [unwired: 1 in]
                n230 = local write "PB Contribution (%)"(w297) -> ()
                n231 = local write "Controller Output (%)"(w289) -> ()
                n232 = local write "Process Variable (%)"(w296) -> ()
                n233 = local write "OP_1 2"(w289) -> ()
                n234 = local write "IOP"(w298) -> ()
                n235 = local write "err"(w300) -> ()
                n236 = local write "SP_1"(w302) -> ()
                n237 = local write "PV_1"(w296) -> ()
                n238 = property on="Waveform Chart" class="WFChart (strict)"("Value"=w301) -> ()  [unwired: 2 in, 2 out]
                n239 = local write "Add Load"(FALSE ("Add Load")) -> ()
                n240 = local write "Tank"(w296) -> ()
                n241 = local write "DOP"(w299) -> ()
              }
            }
          }
          frame "P Mode" {
            # "P Mode"
            n242 = flat-sequence {
              tunnel: [w346] -> w325
              tunnel: [w333] -> w324
              tunnel: w325 -> [w379]
              tunnel: w324 -> [w380]
              tunnel: w323 -> [w378]
              tunnel: w322 -> [w377]
              tunnel: w321 -> [w359]
              tunnel: w320 -> [w376]
              tunnel: w319 -> [_]
              tunnel: w318 -> [_]
              tunnel: [w375] -> w317
              tunnel: w316 -> [_]
              tunnel: [w374] -> w315
              tunnel: [w373] -> w314
              tunnel: [w372] -> w313
              tunnel: w312 -> [w360]
              tunnel: w311 -> [_]
              tunnel: w310 -> [w371]
              tunnel: w309 -> [w370]
              tunnel: [w369] -> w308
              tunnel: w307 -> [_]
              tunnel: [w362] -> w306
              tunnel: [w361] -> w305
              tunnel: [w355] -> w304
              tunnel: w322 -> [w392]
              tunnel: w317 -> [w390]
              tunnel: w315 -> [w389]
              tunnel: w314 -> [w388]
              tunnel: w313 -> [w387]
              tunnel: w308 -> [w386]
              tunnel: w306 -> [w385]
              tunnel: w305 -> [w384]
              tunnel: w304 -> [w381]
              tunnel: [w381] -> w303
              frame #0 {
                n243 = local read "Process Variable (%)"() -> (w347:dbl)
                n244 = local read "Out Flow (%)"() -> (w350:dbl)
                n245 = local read "Constant Outflow"() -> (w332:bool)
                n246 = local read "Action"() -> (w351:bool)
                n247 = local read "Load"() -> (w329:dbl)
                n248 = local read "qi"() -> (w349:dbl)
                n249 = local read "out1"() -> (w348:dbl)
                n250 = local read "Add Load"() -> (w327:bool)
                n251 = local read "Tank Height  (cms)"() -> (w340:dbl)
                n252 = local read "Max. Inflow (LPH)"() -> (w341:dbl)
                n253 = local read "Area"() -> (w343:dbl)
                n254 = Wait Until Next ms Multiple(millisecond multiple=u32 100) -> ()  [unwired: 1 out]
                n255 = local read "K"() -> (w342:dbl)
                n256 = Boolean To (0,1)(Boolean=w327) -> (0, 1=w326:i16)
                n257 = Boolean To (0,1)(Boolean=w351) -> (0, 1=w333:i16)
                n258 = Boolean To (0,1)(Boolean=w332) -> (0, 1=w331:i16)
                n259 = case shown="0, Default" w331 {
                  frame 1 {
                    n260 = property on="Out Flow (%)" class="Slide (strict)"("DisabledEnum"=T9."Enabled" ("Disabled")) -> ()  [unwired: 2 in, 2 out]
                  }
                  frame 0, Default {
                    n261 = property on="Out Flow (%)" class="Slide (strict)"("DisabledEnum"=T9."Disabled and Grayed Out" ("Disabled")) -> ()  [unwired: 2 in, 2 out]
                  }
                }
                n262 = formula code="float dh; float pv; float pv_cm;\n\ndh=(qi-q0)*0.28/A;\npv=(100/h)*dh; \npv1=pv+pv1;\npv_cm=pv1/4;    \n\nif (flow==0) {\nq0=K*A*(sqrt(2*0.098*pv_cm)/0.28);\n}\n\nif (act==0){\nqi=qimax-(out*qimax/100);}\nelse{\nqi=out*qimax/100;    \n}\n\nif (add==1){\npv1=pv1+load;}"("qi"=w349, "act"=w333, "q0"=w350, "out"=w348, "pv1"=w347, "A"=w343, "K"=w342, "qimax"=w341, "h"=w340, "flow"=w331, "add"=w326, "load"=w329) -> ("pv1"=w330:dbl, "qi"=w339:dbl, "q0"=w336:dbl, "dh"=w334:dbl)
                n263 = local write "dh"(w334) -> ()
                n264 = local write "qi"(w339) -> ()
                n265 = In Range and Coerce(upper limit=100.0, x=w336, lower limit=0.0) -> (coerced(x)=w335:dbl)  [unwired: 1 out]
                n266 = local write "Out Flow (%)"(w335) -> ()
                n267 = In Range and Coerce(upper limit=100.0, x=w330, lower limit=0.0) -> (coerced(x)=w346:dbl)  [unwired: 1 out]
              }
              frame #1 {
                n268 = Wait Until Next ms Multiple(millisecond multiple=u32 100) -> ()  [unwired: 1 out]
                n269 = formula code="float kp; \n\nif (PV==1){\npv1=PV1;\n}\n\nif (act==1) {\nerror=sp1-pv1;}\nelse{\nerror=pv1-sp1;\n}\n\nkp=100/PB; \npop=kp*error;\n\nout=pop+bias;\nif (AM==1)\n{\nout=OP;\n}"("sp1"=w377, "pv1"=w379, "act"=w380, "AM"=w376, "OP"=w378, "bias"=w360, "PV"=w371, "PV1"=w370, "PB"=w359) -> ("out"=w356:dbl, "error"=w375:dbl, "iop"=w373:dbl, "dop"=w374:dbl, "pop"=w372:dbl, "pv1"=w369:dbl)
                n270 = property on="Array" class="Arr (strict)"() -> ("Value"=w363:dbl[])  [unwired: 2 in, 2 out]
                n271 = local read "Time Lag (s)"() -> (w364:u32)
                n272 = Rotate 1D Array(1:w363, 2:1 ("n")) -> (0:w366:dbl[])
                n273 = Decrement(x=w364) -> (x-1=w365:u32)
                n274 = In Range and Coerce(upper limit=100.0, x=w356, lower limit=0.0) -> (coerced(x)=w355:dbl)  [unwired: 1 out]
                n275 = Replace Array Subset(array=w366, new element=w355, index=0) -> (w362:dbl[])
                n276 = Index Array(array=w362, index=w365) -> (element=w361:dbl)
              }
              frame #2 {
                n277 = Wait Until Next ms Multiple(millisecond multiple=u32 100) -> ()  [unwired: 1 out]
                n278 = local write "out1"(w384) -> ()
                n279 = property on="Array" class="Arr (strict)"("Value"=w385) -> ()  [unwired: 2 in, 2 out]
                n280 = Bundle("Set Point (%)"=w392, "pv1"=w386, "upper limit"=w381) -> (w391:T10)  [unwired: 1 in]
                n281 = local write "PB Contribution (%)"(w387) -> ()
                n282 = local write "Controller Output (%)"(w381) -> ()
                n283 = local write "Process Variable (%)"(w386) -> ()
                n284 = local write "OP_1 2"(w381) -> ()
                n285 = local write "IOP"(w388) -> ()
                n286 = local write "err"(w390) -> ()
                n287 = local write "SP_1"(w392) -> ()
                n288 = local write "PV_1"(w386) -> ()
                n289 = property on="Waveform Chart" class="WFChart (strict)"("Value"=w391) -> ()  [unwired: 2 in, 2 out]
                n290 = local write "Add Load"(FALSE ("Add Load")) -> ()
                n291 = local write "Tank"(w386) -> ()
                n292 = local write "DOP"(w389) -> ()
              }
            }
          }
          frame "PI Mode" {
            # "PI Mode"
            n293 = flat-sequence {
              tunnel: [w436] -> w416
              tunnel: [w423] -> w415
              tunnel: w416 -> [w474]
              tunnel: w415 -> [w475]
              tunnel: w414 -> [w473]
              tunnel: w413 -> [w472]
              tunnel: w412 -> [w471]
              tunnel: w411 -> [w470]
              tunnel: w410 -> [w469]
              tunnel: w409 -> [w468]
              tunnel: [w467] -> w408
              tunnel: w407 -> [w466]
              tunnel: [w465] -> w406
              tunnel: [w464] -> w405
              tunnel: [w463] -> w404
              tunnel: [w462] -> w403
              tunnel: w402 -> [w461]
              tunnel: w401 -> [w460]
              tunnel: w400 -> [w459]
              tunnel: w399 -> [w458]
              tunnel: [w457] -> w398
              tunnel: w397 -> [w456]
              tunnel: [w449] -> w396
              tunnel: [w448] -> w395
              tunnel: [w444] -> w394
              tunnel: w413 -> [w487]
              tunnel: w408 -> [w485]
              tunnel: w406 -> [w484]
              tunnel: w405 -> [w483]
              tunnel: w404 -> [w482]
              tunnel: w403 -> [w481]
              tunnel: w398 -> [w480]
              tunnel: w396 -> [w479]
              tunnel: w395 -> [w478]
              tunnel: w394 -> [w476]
              tunnel: [w476] -> w393
              frame #0 {
                n294 = local read "Process Variable (%)"() -> (w437:dbl)
                n295 = local read "Out Flow (%)"() -> (w440:dbl)
                n296 = local read "Constant Outflow"() -> (w422:bool)
                n297 = local read "Action"() -> (w441:bool)
                n298 = local read "Add Load"() -> (w418:bool)
                n299 = local read "qi"() -> (w439:dbl)
                n300 = local read "out1"() -> (w438:dbl)
                n301 = local read "Load"() -> (w417:dbl)
                n302 = local read "Tank Height  (cms)"() -> (w430:dbl)
                n303 = local read "Max. Inflow (LPH)"() -> (w431:dbl)
                n304 = local read "Area"() -> (w433:dbl)
                n305 = local read "K"() -> (w432:dbl)
                n306 = Boolean To (0,1)(Boolean=w422) -> (0, 1=w421:i16)
                n307 = Boolean To (0,1)(Boolean=w418) -> (0, 1=w419:i16)
                n308 = Boolean To (0,1)(Boolean=w441) -> (0, 1=w423:i16)
                n309 = case shown="0, Default" w421 {
                  frame 1 {
                    n310 = property on="Out Flow (%)" class="Slide (strict)"("DisabledEnum"=T9."Enabled" ("Disabled")) -> ()  [unwired: 2 in, 2 out]
                  }
                  frame 0, Default {
                    n311 = property on="Out Flow (%)" class="Slide (strict)"("DisabledEnum"=T9."Disabled and Grayed Out" ("Disabled")) -> ()  [unwired: 2 in, 2 out]
                  }
                }
                n312 = formula code="float dh; float pv; float pv_cm;\n\ndh=(qi-q0)*0.28/A;\npv=(100/h)*dh; \npv1=pv+pv1;\npv_cm=pv1/4;    \n\nif (flow==0) {\nq0=K*A*(sqrt(2*0.098*pv_cm)/0.28);\n}\n\nif (act==0){\nqi=qimax-(out*qimax/100);}\nelse{\nqi=out*qimax/100;    \n}\n\nif (add==1){\npv1=pv1+load;}"("qi"=w439, "act"=w423, "q0"=w440, "out"=w438, "pv1"=w437, "A"=w433, "K"=w432, "qimax"=w431, "h"=w430, "flow"=w421, "add"=w419, "load"=w417) -> ("pv1"=w420:dbl, "qi"=w429:dbl, "q0"=w426:dbl, "dh"=w424:dbl)
                n313 = local write "dh"(w424) -> ()
                n314 = local write "qi"(w429) -> ()
                n315 = In Range and Coerce(upper limit=100.0, x=w426, lower limit=0.0) -> (coerced(x)=w425:dbl)  [unwired: 1 out]
                n316 = local write "Out Flow (%)"(w425) -> ()
                n317 = In Range and Coerce(upper limit=100.0, x=w420, lower limit=0.0) -> (coerced(x)=w436:dbl)  [unwired: 1 out]
              }
              frame #1 {
                n318 = formula code="float kp; float ibias;\nif (PV==1){\npv1=PV1;\n}\nif (act==1) {\nerror=sp1-pv1;\n}\nelse {\nerror=pv1-sp1;\n}\nkp=100/PB; \npop=kp*error;\niop=pop/IT;\n\nif (AM==1)\n{\nout=OP;\nif (Bump==1){\nibias=out-pop;\n}\n}\nelse {\nif (Rst==1 && (OP>=100 || OP<=0)) {\nibias=bias;\n}\nelse{\nibias=bias+iop;\n}\nout=pop+iop+ibias;\n}"("sp1"=w472, "pv1"=w474, "act"=w475, "AM"=w470, "OP"=w473, "PB"=w471, "IT"=w469, "DT"=w468, "err"=w466, "bias"=w461, "Bump"=w460, "PV"=w459, "PV1"=w458, "Rst"=w456) -> ("out"=w445:dbl, "error"=w467:dbl, "iop"=w464:dbl, "dop"=w465:dbl, "pop"=w463:dbl, "ibias"=w462:dbl, "pv1"=w457:dbl)
                n319 = property on="Array" class="Arr (strict)"() -> ("Value"=w450:dbl[])  [unwired: 2 in, 2 out]
                n320 = local read "Time Lag (s)"() -> (w451:u32)
                n321 = Rotate 1D Array(1:w450, 2:1 ("n")) -> (0:w453:dbl[])
                n322 = Decrement(x=w451) -> (x-1=w452:u32)
                n323 = In Range and Coerce(upper limit=100.0, x=w445, lower limit=0.0) -> (coerced(x)=w444:dbl)  [unwired: 1 out]
                n324 = Replace Array Subset(array=w453, new element=w444, index=0) -> (w449:dbl[])
                n325 = Index Array(array=w449, index=w452) -> (element=w448:dbl)
              }
              frame #2 {
                n326 = local write "out1"(w478) -> ()
                n327 = property on="Array" class="Arr (strict)"("Value"=w479) -> ()  [unwired: 2 in, 2 out]
                n328 = Bundle("Set Point (%)"=w487, "pv1"=w480, "upper limit"=w476) -> (w486:T10)  [unwired: 1 in]
                n329 = local write "PB Contribution (%)"(w482) -> ()
                n330 = local write "Controller Output (%)"(w476) -> ()
                n331 = local write "Process Variable (%)"(w480) -> ()
                n332 = local write "OP_1 2"(w476) -> ()
                n333 = local write "IOP"(w483) -> ()
                n334 = local write "err"(w485) -> ()
                n335 = local write "SP_1"(w487) -> ()
                n336 = local write "PV_1"(w480) -> ()
                n337 = property on="Waveform Chart" class="WFChart (strict)"("Value"=w486) -> ()  [unwired: 2 in, 2 out]
                n338 = local write "Add Load"(FALSE ("Add Load")) -> ()
                n339 = local write "Tank"(w480) -> ()
                n340 = local write "Bias (%)"(w481) -> ()
                n341 = local write "DOP"(w484) -> ()
              }
            }
          }
          frame "PD Mode" {
            # "PD Mode"
            n342 = flat-sequence {
              tunnel: [w530] -> w510
              tunnel: [w517] -> w509
              tunnel: w510 -> [w567]
              tunnel: w509 -> [w568]
              tunnel: w508 -> [w566]
              tunnel: w507 -> [w565]
              tunnel: w506 -> [w564]
              tunnel: w505 -> [w563]
              tunnel: w504 -> [w562]
              tunnel: w503 -> [w561]
              tunnel: [w560] -> w502
              tunnel: w501 -> [w559]
              tunnel: [w558] -> w500
              tunnel: [w557] -> w499
              tunnel: [w556] -> w498
              tunnel: w497 -> [w555]
              tunnel: w496 -> [w554]
              tunnel: w495 -> [w553]
              tunnel: w494 -> [w552]
              tunnel: [w551] -> w493
              tunnel: w492 -> [w550]
              tunnel: [w543] -> w491
              tunnel: [w542] -> w490
              tunnel: [w538] -> w489
              tunnel: w507 -> [w579]
              tunnel: w502 -> [w577]
              tunnel: w500 -> [w576]
              tunnel: w499 -> [w575]
              tunnel: w498 -> [w574]
              tunnel: w493 -> [w573]
              tunnel: w491 -> [w572]
              tunnel: w490 -> [w571]
              tunnel: w489 -> [w569]
              tunnel: [w569] -> w488
              frame #0 {
                n343 = local read "Process Variable (%)"() -> (w531:dbl)
                n344 = local read "Out Flow (%)"() -> (w534:dbl)
                n345 = local read "Constant Outflow"() -> (w516:bool)
                n346 = local read "Action"() -> (w535:bool)
                n347 = local read "Add Load"() -> (w512:bool)
                n348 = local read "qi"() -> (w533:dbl)
                n349 = local read "out1"() -> (w532:dbl)
                n350 = local read "Load"() -> (w511:dbl)
                n351 = local read "Tank Height  (cms)"() -> (w524:dbl)
                n352 = local read "Max. Inflow (LPH)"() -> (w525:dbl)
                n353 = local read "Area"() -> (w527:dbl)
                n354 = local read "K"() -> (w526:dbl)
                n355 = Boolean To (0,1)(Boolean=w516) -> (0, 1=w515:i16)
                n356 = Boolean To (0,1)(Boolean=w512) -> (0, 1=w513:i16)
                n357 = Boolean To (0,1)(Boolean=w535) -> (0, 1=w517:i16)
                n358 = case shown="0, Default" w515 {
                  frame 1 {
                    n359 = property on="Out Flow (%)" class="Slide (strict)"("DisabledEnum"=T9."Enabled" ("Disabled")) -> ()  [unwired: 2 in, 2 out]
                  }
                  frame 0, Default {
                    n360 = property on="Out Flow (%)" class="Slide (strict)"("DisabledEnum"=T9."Disabled and Grayed Out" ("Disabled")) -> ()  [unwired: 2 in, 2 out]
                  }
                }
                n361 = formula code="float dh; float pv; float pv_cm;\n\ndh=(qi-q0)*0.28/A;\npv=(100/h)*dh; \npv1=pv+pv1;\npv_cm=pv1/4;    \n\nif (flow==0) {\nq0=K*A*(sqrt(2*0.098*pv_cm)/0.28);\n}\n\nif (act==0){\nqi=qimax-(out*qimax/100);}\nelse{\nqi=out*qimax/100;    \n}\n\nif (add==1){\npv1=pv1+load;}"("qi"=w533, "act"=w517, "q0"=w534, "out"=w532, "pv1"=w531, "A"=w527, "K"=w526, "qimax"=w525, "h"=w524, "flow"=w515, "add"=w513, "load"=w511) -> ("pv1"=w514:dbl, "qi"=w523:dbl, "q0"=w520:dbl, "dh"=w518:dbl)
                n362 = local write "dh"(w518) -> ()
                n363 = local write "qi"(w523) -> ()
                n364 = In Range and Coerce(upper limit=100.0, x=w520, lower limit=0.0) -> (coerced(x)=w519:dbl)  [unwired: 1 out]
                n365 = local write "Out Flow (%)"(w519) -> ()
                n366 = In Range and Coerce(upper limit=100.0, x=w514, lower limit=0.0) -> (coerced(x)=w530:dbl)  [unwired: 1 out]
              }
              frame #1 {
                n367 = formula code="float kp; float de;\nif (PV==1){\npv1=PV1;\n}\nif (act==1) {\nerror=sp1-pv1;\n}\nelse {\nerror=pv1-sp1;\n}\nkp=100/PB; \npop=kp*error;\nde=error-err; \ndop=kp*DT*de;\nif (AM==1){\nout=OP;}\nelse{\nout=pop+dop+bias;\n}"("sp1"=w565, "pv1"=w567, "act"=w568, "AM"=w563, "OP"=w566, "PB"=w564, "IT"=w562, "DT"=w561, "err"=w559, "bias"=w555, "Bump"=w554, "PV"=w553, "PV1"=w552, "Rst"=w550) -> ("out"=w539:dbl, "error"=w560:dbl, "iop"=w557:dbl, "dop"=w558:dbl, "pop"=w556:dbl, "pv1"=w551:dbl)
                n368 = property on="Array" class="Arr (strict)"() -> ("Value"=w544:dbl[])  [unwired: 2 in, 2 out]
                n369 = local read "Time Lag (s)"() -> (w545:u32)
                n370 = Rotate 1D Array(1:w544, 2:1 ("n")) -> (0:w547:dbl[])
                n371 = Decrement(x=w545) -> (x-1=w546:u32)
                n372 = In Range and Coerce(upper limit=100.0, x=w539, lower limit=0.0) -> (coerced(x)=w538:dbl)  [unwired: 1 out]
                n373 = Replace Array Subset(array=w547, new element=w538, index=0) -> (w543:dbl[])
                n374 = Index Array(array=w543, index=w546) -> (element=w542:dbl)
              }
              frame #2 {
                n375 = local write "out1"(w571) -> ()
                n376 = property on="Array" class="Arr (strict)"("Value"=w572) -> ()  [unwired: 2 in, 2 out]
                n377 = Bundle("Set Point (%)"=w579, "pv1"=w573, "upper limit"=w569) -> (w578:T10)  [unwired: 1 in]
                n378 = local write "PB Contribution (%)"(w574) -> ()
                n379 = local write "Controller Output (%)"(w569) -> ()
                n380 = local write "Process Variable (%)"(w573) -> ()
                n381 = local write "OP_1 2"(w569) -> ()
                n382 = local write "IOP"(w575) -> ()
                n383 = local write "err"(w577) -> ()
                n384 = local write "SP_1"(w579) -> ()
                n385 = local write "PV_1"(w573) -> ()
                n386 = property on="Waveform Chart" class="WFChart (strict)"("Value"=w578) -> ()  [unwired: 2 in, 2 out]
                n387 = local write "Add Load"(FALSE ("Add Load")) -> ()
                n388 = local write "Tank"(w573) -> ()
                n389 = local write "DOP"(w576) -> ()
              }
            }
          }
          frame "PID Mode", Default {
            # "PID Mode"
            n390 = flat-sequence {
              tunnel: [w623] -> w603
              tunnel: [w610] -> w602
              tunnel: w603 -> [w661]
              tunnel: w602 -> [w662]
              tunnel: w601 -> [w660]
              tunnel: w600 -> [w659]
              tunnel: w599 -> [w658]
              tunnel: w598 -> [w657]
              tunnel: w597 -> [w656]
              tunnel: w596 -> [w655]
              tunnel: [w654] -> w595
              tunnel: w594 -> [w653]
              tunnel: [w652] -> w593
              tunnel: [w651] -> w592
              tunnel: [w650] -> w591
              tunnel: [w649] -> w590
              tunnel: w589 -> [w648]
              tunnel: w588 -> [w647]
              tunnel: w587 -> [w646]
              tunnel: w586 -> [w645]
              tunnel: [w644] -> w585
              tunnel: w584 -> [w643]
              tunnel: [w636] -> w583
              tunnel: [w635] -> w582
              tunnel: [w631] -> w581
              tunnel: w600 -> [w674]
              tunnel: w595 -> [w672]
              tunnel: w593 -> [w671]
              tunnel: w592 -> [w670]
              tunnel: w591 -> [w669]
              tunnel: w590 -> [w668]
              tunnel: w585 -> [w667]
              tunnel: w583 -> [w666]
              tunnel: w582 -> [w665]
              tunnel: w581 -> [w663]
              tunnel: [w663] -> w580
              frame #0 {
                n391 = local read "Process Variable (%)"() -> (w624:dbl)
                n392 = local read "Out Flow (%)"() -> (w627:dbl)
                n393 = local read "Constant Outflow"() -> (w609:bool)
                n394 = local read "Action"() -> (w628:bool)
                n395 = local read "Add Load"() -> (w605:bool)
                n396 = local read "qi"() -> (w626:dbl)
                n397 = local read "out1"() -> (w625:dbl)
                n398 = local read "Load"() -> (w604:dbl)
                n399 = local read "Tank Height  (cms)"() -> (w617:dbl)
                n400 = local read "Max. Inflow (LPH)"() -> (w618:dbl)
                n401 = local read "Area"() -> (w620:dbl)
                n402 = local read "K"() -> (w619:dbl)
                n403 = Boolean To (0,1)(Boolean=w609) -> (0, 1=w608:i16)
                n404 = Boolean To (0,1)(Boolean=w605) -> (0, 1=w606:i16)
                n405 = Boolean To (0,1)(Boolean=w628) -> (0, 1=w610:i16)
                n406 = case shown="0, Default" w608 {
                  frame 1 {
                    n407 = property on="Out Flow (%)" class="Slide (strict)"("DisabledEnum"=T9."Enabled" ("Disabled")) -> ()  [unwired: 2 in, 2 out]
                  }
                  frame 0, Default {
                    n408 = property on="Out Flow (%)" class="Slide (strict)"("DisabledEnum"=T9."Disabled and Grayed Out" ("Disabled")) -> ()  [unwired: 2 in, 2 out]
                  }
                }
                n409 = formula code="float dh; float pv; float pv_cm;\n\ndh=(qi-q0)*0.28/A;\npv=(100/h)*dh; \npv1=pv+pv1;\npv_cm=pv1/4;    \n\nif (flow==0) {\nq0=K*A*(sqrt(2*0.098*pv_cm)/0.28);\n}\n\nif (act==0){\nqi=qimax-(out*qimax/100);}\nelse{\nqi=out*qimax/100;    \n}\n\nif (add==1){\npv1=pv1+load;}"("qi"=w626, "act"=w610, "q0"=w627, "out"=w625, "pv1"=w624, "A"=w620, "K"=w619, "qimax"=w618, "h"=w617, "flow"=w608, "add"=w606, "load"=w604) -> ("pv1"=w607:dbl, "qi"=w616:dbl, "q0"=w613:dbl, "dh"=w611:dbl)
                n410 = local write "dh"(w611) -> ()
                n411 = local write "qi"(w616) -> ()
                n412 = In Range and Coerce(upper limit=100.0, x=w613, lower limit=0.0) -> (coerced(x)=w612:dbl)  [unwired: 1 out]
                n413 = local write "Out Flow (%)"(w612) -> ()
                n414 = In Range and Coerce(upper limit=100.0, x=w607, lower limit=0.0) -> (coerced(x)=w623:dbl)  [unwired: 1 out]
              }
              frame #1 {
                n415 = formula code="float kp; float de; float ibias;\nif (PV==1){\npv1=PV1;\n}\nif (act==1) {\nerror=sp1-pv1;\n}\nelse {\nerror=pv1-sp1;\n}\nkp=100/PB; \npop=kp*error;\niop=pop/IT;\nde=error-err; \ndop=kp*DT*de;\nif (AM==1)\n{\nout=OP;\nif (Bump==1){\nibias=out-(pop+dop);\n}\n}\nelse {\nif (Rst==1 && (OP>=100 || OP<=0)) {\nibias=bias;\n}\nelse{\nibias=bias+iop;\n}\nout=pop+iop+dop+ibias;\n}"("sp1"=w659, "pv1"=w661, "act"=w662, "AM"=w657, "OP"=w660, "PB"=w658, "IT"=w656, "DT"=w655, "err"=w653, "bias"=w648, "Bump"=w647, "PV"=w646, "PV1"=w645, "Rst"=w643) -> ("out"=w632:dbl, "error"=w654:dbl, "iop"=w651:dbl, "dop"=w652:dbl, "pop"=w650:dbl, "ibias"=w649:dbl, "pv1"=w644:dbl)
                n416 = property on="Array" class="Arr (strict)"() -> ("Value"=w637:dbl[])  [unwired: 2 in, 2 out]
                n417 = local read "Time Lag (s)"() -> (w638:u32)
                n418 = Rotate 1D Array(1:w637, 2:1 ("n")) -> (0:w640:dbl[])
                n419 = Decrement(x=w638) -> (x-1=w639:u32)
                n420 = In Range and Coerce(upper limit=100.0, x=w632, lower limit=0.0) -> (coerced(x)=w631:dbl)  [unwired: 1 out]
                n421 = Replace Array Subset(array=w640, new element=w631, index=0) -> (w636:dbl[])
                n422 = Index Array(array=w636, index=w639) -> (element=w635:dbl)
              }
              frame #2 {
                n423 = local write "out1"(w665) -> ()
                n424 = property on="Array" class="Arr (strict)"("Value"=w666) -> ()  [unwired: 2 in, 2 out]
                n425 = Bundle("Set Point (%)"=w674, "pv1"=w667, "upper limit"=w663) -> (w673:T10)  [unwired: 1 in]
                n426 = local write "PB Contribution (%)"(w669) -> ()
                n427 = local write "Controller Output (%)"(w663) -> ()
                n428 = local write "Process Variable (%)"(w667) -> ()
                n429 = local write "OP_1 2"(w663) -> ()
                n430 = local write "IOP"(w670) -> ()
                n431 = local write "err"(w672) -> ()
                n432 = local write "SP_1"(w674) -> ()
                n433 = local write "Add Load"(FALSE ("Add Load")) -> ()
                n434 = local write "PV_1"(w667) -> ()
                n435 = property on="Waveform Chart" class="WFChart (strict)"("Value"=w673) -> ()  [unwired: 2 in, 2 out]
                n436 = local write "Tank"(w667) -> ()
                n437 = local write "Bias (%)"(w668) -> ()
                n438 = local write "DOP"(w671) -> ()
              }
            }
          }
        }
        n439 = case shown="1, Default" w131 {
          frame 1, Default {
            n440 = property on="Controller Output (%)" class="Slide (strict)"("DisabledEnum"=T9."Enabled" ("Disabled")) -> ()  [unwired: 2 in, 2 out]
          }
          frame 0 {
            n441 = property on="Controller Output (%)" class="Slide (strict)"("DisabledEnum"=T9."Disabled and Grayed Out" ("Disabled")) -> ()  [unwired: 2 in, 2 out]
          }
        }
        n442 = case shown="0, Default" w127 {
          frame 0, Default {
            w171 = T9."Enabled" ("Disabled")
            n443 = property on="Add Load" class="Bool (strict)"("DisabledEnum"=w171) -> ()  [unwired: 2 in, 2 out]
            n444 = property on="Load" class="Slide (strict)"("DisabledEnum"=w171) -> ()  [unwired: 2 in, 2 out]
            n445 = property on="Process Variable (%)" class="Slide (strict)"("DisabledEnum"=T9."Disabled and Grayed Out" ("Disabled")) -> ()  [unwired: 2 in, 2 out]
          }
          frame 1 {
            w173 = T9."Disabled and Grayed Out" ("Disabled")
            n446 = property on="Process Variable (%)" class="Slide (strict)"("DisabledEnum"=T9."Enabled" ("Disabled")) -> ()  [unwired: 2 in, 2 out]
            n447 = property on="Add Load" class="Bool (strict)"("DisabledEnum"=w173) -> ()  [unwired: 2 in, 2 out]
            n448 = property on="Load" class="Slide (strict)"("DisabledEnum"=w173) -> ()  [unwired: 2 in, 2 out]
          }
        }
        n449 = property on="Experiment Selection" class="Ring (strict)"("DisabledEnum"=w123) -> ()  [unwired: 2 in, 2 out]
        n450 = property on="Run" class="Bool (strict)"("DisabledEnum"=w123) -> ()  [unwired: 2 in, 2 out]
        n451 = property on="Home" class="Bool (strict)"("DisabledEnum"=w123) -> ()  [unwired: 2 in, 2 out]
        n452 = property on="Single Step" class="Bool (strict)"("DisabledEnum"=w123) -> ()  [unwired: 2 in, 2 out]
        n453 = property on="Action" class="Bool (strict)"("DisabledEnum"=w116) -> ()  [unwired: 2 in, 2 out]
        n454 = property on="Radio Buttons" class="RadioBtnsControl (strict)"("DisabledEnum"=w116) -> ()  [unwired: 2 in, 2 out]
        n455 = property on="Pause" class="Bool (strict)"("DisabledEnum"=w124) -> ()  [unwired: 2 in, 2 out]
        n456 = property on="Stop" class="Bool (strict)"("DisabledEnum"=w124) -> ()  [unwired: 2 in, 2 out]
        n457 = property on="Log Button" class="Bool (strict)"("DisabledEnum"=w124) -> ()  [unwired: 2 in, 2 out]
        n458 = local read "Stop Flag"() -> (w117:bool)
        n459 = local read "Pause"() -> (w114:bool)
        n460 = local read "Stop"() -> (w119:bool)
        n461 = Compound Arithmetic op=OR(w119, w117, w114) -> (w118:bool)
        n462 = case shown="False" w118 {
          frame False {
            n463 = Wait Until Next ms Multiple(millisecond multiple=u32 1000) -> ()  [unwired: 1 out]
          }
          frame True {
          }
        }
        n464 = Select(t=T2."Pause", s=w114, f=T2."Play") -> (s? t:f=w126:T2)
        n465 = Select(t=T2."Stop", s=w118, f=w126) -> (s? t:f=w125:T2)
        n466 = case shown="True" w114 {
          frame False {
          }
          frame True {
            w167 = T9."Enabled" ("Disabled")
            n467 = property on="Run" class="Bool (strict)"("DisabledEnum"=w167) -> ()  [unwired: 2 in, 2 out]
            n468 = property on="Single Step" class="Bool (strict)"("DisabledEnum"=w167) -> ()  [unwired: 2 in, 2 out]
            n469 = local write "Run"(FALSE ("Play Button")) -> ()
            n470 = property on="Run" class="Bool (strict)"("Colors [4]"=cluster{u32, u32}[] [{16777216, 16777215}]) -> ()  [unwired: 2 in, 2 out]
            n471 = property on="Pause" class="Bool (strict)"("DisabledEnum"=T9."Disabled" ("Disabled")) -> ()  [unwired: 2 in, 2 out]
          }
        }
        n472 = local read "Log Button"() -> (w139:bool)
        n473 = case shown="True" w139 {
          tunnel: w115 -> [_ w183]
          frame False {
            n474 = local read "Log Count"() -> (w179:dbl)
            n475 = local read "Save Log"() -> (w176:bool)
            n476 = property on="Log" class="Bool (strict)"("Blinking"=FALSE) -> ()  [unwired: 2 in, 2 out]
            n477 = Equal?(x=w179, y=0.0) -> (x = y?=w178:bool)
            n478 = case shown="True" w176 {
              frame False {
              }
              frame True {
                n479 = invoke on="Table" class="Tbl (strict)" method="Export Data to Excel"() -> ()  [unwired: 3 in, 3 out]
                n480 = local write "Save Log"(FALSE ("Save")) -> ()
              }
            }
            n481 = case shown="False" w178 {
              frame False {
                w181 = T9."Enabled" ("Disabled")
                n482 = property on="Clear" class="Bool (strict)"("DisabledEnum"=w181) -> ()  [unwired: 2 in, 2 out]
                n483 = property on="Save Log" class="Bool (strict)"("DisabledEnum"=w181) -> ()  [unwired: 2 in, 2 out]
              }
              frame True {
                w182 = T9."Disabled" ("Disabled")
                n484 = property on="Clear" class="Bool (strict)"("DisabledEnum"=w182) -> ()  [unwired: 2 in, 2 out]
                n485 = property on="Save Log" class="Bool (strict)"("DisabledEnum"=w182) -> ()  [unwired: 2 in, 2 out]
              }
            }
          }
          frame True {
            w185 = T9."Disabled" ("Disabled")
            w200 = i16 1 ("precision (6)")
            n486 = disable-structure shown="Disabled" {
              frame Disabled {
                n487 = local read "Controller Output (%)"() -> ()  [unwired: 1 out]
              }
              frame Enabled {
              }
            }
            n488 = local read "Process Variable (%)"() -> (w196:dbl)
            n489 = property on="Log" class="Bool (strict)"("Blinking"=TRUE) -> ()  [unwired: 2 in, 2 out]
            n490 = local read "Set Point (%)"() -> (w195:dbl)
            n491 = local read "Log Count"() -> (w184:dbl)
            n492 = local read "PB %"() -> (w197:dbl)
            n493 = local read "DT s"() -> (w199:dbl)
            n494 = local read "IT s"() -> (w198:dbl)
            n495 = property on="Clear" class="Bool (strict)"("DisabledEnum"=w185) -> ()  [unwired: 2 in, 2 out]
            n496 = property on="Save Log" class="Bool (strict)"("DisabledEnum"=w185) -> ()  [unwired: 2 in, 2 out]
            n497 = Increment(x=w184) -> (x+1=w187:dbl)
            n498 = local write "Log Count"(w187) -> ()
            n499 = Subtract(x=w187, y=9.0) -> (x-y=w191:dbl)
            n500 = Number To Decimal String(number=w187, width (-)=w200) -> (decimal integer string=w205:string)
            n501 = Number To Fractional String(number=w195, precision (6)=w200) -> (F-format string=w206:string)  [unwired: 2 in]
            n502 = Number To Fractional String(number=w196, precision (6)=w200) -> (F-format string=w204:string)  [unwired: 2 in]
            n503 = Number To Fractional String(number=w183, precision (6)=w200) -> (F-format string=w207:string)  [unwired: 2 in]
            n504 = Number To Fractional String(number=w197, precision (6)=w200) -> (F-format string=w203:string)  [unwired: 2 in]
            n505 = Number To Fractional String(number=w198, precision (6)=w200) -> (F-format string=w201:string)  [unwired: 2 in]
            n506 = Number To Fractional String(number=w199, precision (6)=w200) -> (F-format string=w202:string)  [unwired: 2 in]
            n507 = Bundle(w191, "X Index"=0) -> (w189:cluster{dbl, "X Index":i32})  [unwired: 1 in]
            n508 = Get Date/Time String(want seconds? (F)=TRUE) -> (time string=w193:string)  [unwired: 2 in, 1 out]
            n509 = property on="Table" class="Tbl (strict)"("Index Values"=w189) -> ()  [unwired: 2 in, 2 out]
            n510 = invoke on="Table" class="Tbl (strict)" method="Set Cell Value"("X Index"=1, "Y Index"=w184, "Value"=w205) -> ()  [unwired: 3 in, 6 out]
            n511 = invoke on="Table" class="Tbl (strict)" method="Set Cell Value"("X Index"=2, "Y Index"=w184, "Value"=w206) -> ()  [unwired: 3 in, 6 out]
            n512 = invoke on="Table" class="Tbl (strict)" method="Set Cell Value"("X Index"=3, "Y Index"=w184, "Value"=w204) -> ()  [unwired: 3 in, 6 out]
            n513 = invoke on="Table" class="Tbl (strict)" method="Set Cell Value"("X Index"=4, "Y Index"=w184, "Value"=w207) -> ()  [unwired: 3 in, 6 out]
            n514 = invoke on="Table" class="Tbl (strict)" method="Set Cell Value"("X Index"=5, "Y Index"=w184, "Value"=w203) -> ()  [unwired: 3 in, 6 out]
            n515 = invoke on="Table" class="Tbl (strict)" method="Set Cell Value"("X Index"=6, "Y Index"=w184, "Value"=w201) -> ()  [unwired: 3 in, 6 out]
            n516 = invoke on="Table" class="Tbl (strict)" method="Set Cell Value"("X Index"=7, "Y Index"=w184, "Value"=w202) -> ()  [unwired: 3 in, 6 out]
            n517 = invoke on="Table" class="Tbl (strict)" method="Set Cell Value"("X Index"=0, "Y Index"=w184, "Value"=w193) -> ()  [unwired: 3 in, 6 out]
          }
        }
      }
      frame "Stop" {
        n518 = local read "Stop Flag"() -> (w675:bool)
        n519 = local read "Pause"() -> (w680:bool)
        n520 = case shown="True" w680 {
          tunnel: [T5."Play" T5."Pause"] -> w679
          frame False {
          }
          frame True {
          }
        }
        n521 = case shown="True" w675 {
          frame False {
            n522 = local write "Stop"(FALSE ("OK Button")) -> ()
            n523 = local write "Bumpless Transfer"(TRUE ("Bumpless Transfer")) -> ()
          }
          frame True {
            w689 = u32 9868950
            w688 = cluster{u32, u32}[] [{16777216, 16777215}] ("Colors [4]")
            n524 = property on="Run" class="Bool (strict)"("BoolText.TextColor"=w689) -> ()  [unwired: 2 in, 2 out]
            n525 = property on="Log Button" class="Bool (strict)"("BoolText.TextColor"=w689) -> ()  [unwired: 2 in, 2 out]
            n526 = property on="Run" class="Bool (strict)"("Colors [4]"=w688) -> ()  [unwired: 2 in, 2 out]
            n527 = property on="Log Button" class="Bool (strict)"("Colors [4]"=w688) -> ()  [unwired: 2 in, 2 out]
          }
        }
        n528 = property on="Log" class="Bool (strict)"("Blinking"=FALSE) -> ()  [unwired: 2 in, 2 out]
        n529 = Select(t=T5."Initialize", s=w675, f=w679) -> (s? t:f=w682:T5)
        n530 = property on="Run" class="Bool (strict)"("BoolText.TextColor"=u32 9868950) -> ()  [unwired: 2 in, 2 out]
        n531 = Wait Until Next ms Multiple(millisecond multiple=u32 10) -> ()  [unwired: 1 out]
        n532 = property on="Pause" class="Bool (strict)"("Colors [4]"=cluster{u32, u32}[] [{16777216, 16777215}]) -> ()  [unwired: 2 in, 2 out]
      }
      frame "Error" {
        n533 = call "Communication Error"() -> ("Retry"=w693:bool)  [unwired: 10 in, 1 out]
        n534 = Select(t=T5."Select Exp", s=w693, f=T5."MainPage") -> (s? t:f=w692:T5)
      }
      frame "Pause" {
        w697 = T9."Enabled" ("Disabled")
        n535 = property on="Run" class="Bool (strict)"("BoolText.TextColor"=u32 9868950) -> ()  [unwired: 2 in, 2 out]
        n536 = property on="Single Step" class="Bool (strict)"("DisabledEnum"=w697) -> ()  [unwired: 2 in, 2 out]
        n537 = property on="Run" class="Bool (strict)"("DisabledEnum"=w697) -> ()  [unwired: 2 in, 2 out]
        n538 = flat-sequence {
          tunnel: [w706] -> w701
          tunnel: [w705] -> w700
          tunnel: [w704] -> w699
          tunnel: w701 -> [w712]
          tunnel: w700 -> [w714]
          tunnel: w699 -> [w713]
          tunnel: [w712] -> w698
          frame #0 {
            n539 = local read "Single Step"() -> (w705:bool)
            n540 = local read "Run"() -> (w704:bool)
            n541 = local read "Stop Flag"() -> (w707:bool)
            n542 = Or(x=w704, y=w705) -> (x .or. y?=w711:bool)
            n543 = Select(t=T5."Play", s=w711, f=T5."Pause") -> (s? t:f=w709:T5)
            n544 = Select(t=T5."Stop", s=w707, f=w709) -> (s? t:f=w706:T5)
          }
          frame #1 {
            n545 = case shown="True" w713 {
              frame False {
              }
              frame True {
                w718 = FALSE ("Pause")
                n546 = local write "Pause"(w718) -> ()
                n547 = local write "Run"(w718) -> ()
                n548 = property on="Pause" class="Bool (strict)"("Colors [4]"=cluster{u32, u32}[] [{16777216, 16777215}]) -> ()  [unwired: 2 in, 2 out]
              }
            }
            n549 = case shown="True" w714 {
              frame False {
              }
              frame True {
                n550 = local write "Single Step"(FALSE ("Pause")) -> ()
                n551 = local write "Pause"(TRUE ("Pause")) -> ()
              }
            }
          }
        }
        n552 = property on="Pause" class="Bool (strict)"("BoolText.TextColor"=u32 9868950) -> ()  [unwired: 2 in, 2 out]
        n553 = local read "Log Button"() -> (w702:bool)
        n554 = property on="Pause" class="Bool (strict)"("Colors [4]"=cluster{u32, u32}[] [{16777216, 32768}]) -> ()  [unwired: 2 in, 2 out]
        n555 = case shown="False" w702 {
          frame False {
            n556 = local read "Log Count"() -> (w721:dbl)
            n557 = Equal?(x=w721, y=0.0) -> (x = y?=w720:bool)
            n558 = case shown="True" w720 {
              frame False {
                w722 = T9."Enabled" ("Disabled")
                n559 = property on="Clear" class="Bool (strict)"("DisabledEnum"=w722) -> ()  [unwired: 2 in, 2 out]
                n560 = property on="Save Log" class="Bool (strict)"("DisabledEnum"=w722) -> ()  [unwired: 2 in, 2 out]
              }
              frame True {
                w724 = T9."Disabled" ("Disabled")
                n561 = property on="Clear" class="Bool (strict)"("Colors [4]"=cluster{u32, u32}[] [{16777216, 16777215}]) -> ()  [unwired: 2 in, 2 out]
                n562 = property on="Clear" class="Bool (strict)"("DisabledEnum"=w724) -> ()  [unwired: 2 in, 2 out]
                n563 = property on="Save Log" class="Bool (strict)"("DisabledEnum"=w724) -> ()  [unwired: 2 in, 2 out]
              }
            }
          }
          frame True {
            w725 = T9."Disabled" ("Disabled")
            n564 = property on="Clear" class="Bool (strict)"("DisabledEnum"=w725) -> ()  [unwired: 2 in, 2 out]
            n565 = property on="Save Log" class="Bool (strict)"("DisabledEnum"=w725) -> ()  [unwired: 2 in, 2 out]
          }
        }
      }
      frame "MainPage" {
        w726 = FALSE ("Previous Button")
        n566 = Current VI's Path() -> (path=w727:path)
        n567 = Open VI Reference(vi path=w727) -> (vi reference=w741:refnum<vi>, error out=w740:errorcluster)  [unwired: 5 in]
        n568 = invoke on="Invoke Node" class="VI" method="FP.Close"(reference=w741, error in=w740) -> (reference out=w739:refnum<vi>, error out=w738:errorcluster)  [unwired: 1 in, 1 out]
        n569 = Close Reference(reference=w739, error in (no error)=w738) -> ()  [unwired: 1 out]
        n570 = local write "Pause"(w726) -> ()
        n571 = local write "Home"(w726) -> ()
        n572 = Open VI Reference(vi path=path "Main.vi") -> (vi reference=w731:refnum<vi>, error out=w728:errorcluster)  [unwired: 2 in, 3 out]
        n573 = invoke class="VI" method="FP.Open"(reference=w731, error in=w728, "Activate"=TRUE) -> (reference out=w729:refnum<vi>, error out=w730:errorcluster)  [unwired: 2 in, 3 out]
        n574 = invoke class="VI" method="Run VI"(reference=w729, error in=w730, "Wait until done"=FALSE, "Auto Dispose Ref"=FALSE) -> (reference out=w736:refnum<vi>, error out=w735:errorcluster)  [unwired: 1 in, 3 out]
        n575 = Close Reference(reference=w736, error in (no error)=w735) -> ()  [unwired: 1 out]
        n576 = Wait Until Next ms Multiple(millisecond multiple=u32 100 ("milliseconds to wait")) -> ()  [unwired: 1 out]
      }
    }
    n577 = Get Date/Time In Seconds() -> (seconds since 1Jan1904=→"current time":timestamp)
    "Enum" <- w8
  }
  n578 = while {
    tunnel: w3 -> [w744]
    stop <- w743 stop-if-true
    n579 = event shown="[38] \"help\": Value Change" {
      selector: w744 -> [_ _ _ _ _ _ _ _ _ _ _ _ _ _ _ _ _ _ _ _ _ _ _ _ _ _ _ _ _ _ _ _ _ _ _ _ _ _ _]
      dyn-events: _ -> [_ _ _ _ _ _ _ _ _ _ _ _ _ _ _ _ _ _ _ _ _ _ _ _ _ _ _ _ _ _ _ _ _ _ _ _ _ _ _]
      timeout: _ -> [_ _ _ _ _ _ _ _ _ _ _ _ _ _ _ _ _ _ _ _ _ _ _ _ _ _ _ _ _ _ _ _ _ _ _ _ _ _ _]
      tunnel: [_ _ _ _ _ _ _ _ _ _ _ _ _ _ _ _ _ _ _ _ _ _ _ _ _ _ _ _ _ _ _ _ _ _ _ _ _ w908 _] -> w743
      tunnel: [_ _ _ _ _ _ _ _ _ _ _ _ _ _ _ _ _ _ _ _ _ _ _ _ _ _ _ _ _ _ _ _ _ _ _ _ w903 _ _] -> _
      tunnel: [_ _ _ _ _ _ _ _ _ _ _ _ _ _ _ _ _ _ _ _ _ _ _ _ _ _ _ _ _ _ _ _ _ _ _ _ _ _ w910] -> _
      event User Event {
        n580 = event-data() -> ()  [unwired: 1 in, 5 out]
      }
      event "Run": Mouse Enter {
        n581 = event-data() -> ()  [unwired: 1 in, 4 out]
        n582 = property on="Run" class="Bool (strict)"() -> ("DisabledEnum"=w746:T9)  [unwired: 2 in, 2 out]
        n583 = Equal?(x=w746, y=T9."Enabled" ("Disabled")) -> (x = y?=w747:bool)
        n584 = case shown="True" w747 {
          frame False {
          }
          frame True {
            n585 = property on="Run" class="Bool (strict)"("BoolText.TextColor"=u32 16448250) -> ()  [unwired: 2 in, 2 out]
            n586 = property on="Run" class="Bool (strict)"("Colors [4]"=cluster{u32, u32}[] [{16777216, 6254465}]) -> ()  [unwired: 2 in, 2 out]
            n587 = call-poly <vilib>:"Set Cursor.vi"("icon"=u16 6) -> ()  [unwired: 9 in, 2 out]
          }
        }
      }
      event "Pause": Mouse Enter {
        n588 = event-data() -> ()  [unwired: 1 in, 4 out]
        n589 = property on="Pause" class="Bool (strict)"() -> ("DisabledEnum"=w752:T9)  [unwired: 2 in, 2 out]
        n590 = Equal?(x=w752, y=T9."Enabled" ("Disabled")) -> (x = y?=w753:bool)
        n591 = case shown="True" w753 {
          frame False {
          }
          frame True {
            n592 = property on="Pause" class="Bool (strict)"("BoolText.TextColor"=u32 16448250) -> ()  [unwired: 2 in, 2 out]
            n593 = property on="Pause" class="Bool (strict)"("Colors [4]"=cluster{u32, u32}[] [{16777216, 6254465}]) -> ()  [unwired: 2 in, 2 out]
            n594 = call-poly <vilib>:"Set Cursor.vi"("icon"=u16 6) -> ()  [unwired: 9 in, 2 out]
          }
        }
      }
      event "Single Step": Mouse Enter {
        n595 = event-data() -> ()  [unwired: 1 in, 4 out]
        n596 = property on="Single Step" class="Bool (strict)"() -> ("DisabledEnum"=w758:T9)  [unwired: 2 in, 2 out]
        n597 = Equal?(x=w758, y=T9."Enabled" ("Disabled")) -> (x = y?=w759:bool)
        n598 = case shown="True" w759 {
          frame False {
          }
          frame True {
            n599 = property on="Single Step" class="Bool (strict)"("BoolText.TextColor"=u32 16448250) -> ()  [unwired: 2 in, 2 out]
            n600 = property on="Single Step" class="Bool (strict)"("Colors [4]"=cluster{u32, u32}[] [{16777216, 6254465}]) -> ()  [unwired: 2 in, 2 out]
            n601 = call-poly <vilib>:"Set Cursor.vi"("icon"=u16 6) -> ()  [unwired: 9 in, 2 out]
          }
        }
      }
      event "Stop": Mouse Enter {
        n602 = event-data() -> ()  [unwired: 1 in, 4 out]
        n603 = property on="Stop" class="Bool (strict)"() -> ("DisabledEnum"=w764:T9)  [unwired: 2 in, 2 out]
        n604 = Equal?(x=w764, y=T9."Enabled" ("Disabled")) -> (x = y?=w765:bool)
        n605 = case shown="True" w765 {
          frame False {
          }
          frame True {
            n606 = property on="Stop" class="Bool (strict)"("BoolText.TextColor"=u32 16448250) -> ()  [unwired: 2 in, 2 out]
            n607 = property on="Stop" class="Bool (strict)"("Colors [4]"=cluster{u32, u32}[] [{16777216, 6254465}]) -> ()  [unwired: 2 in, 2 out]
            n608 = call-poly <vilib>:"Set Cursor.vi"("icon"=u16 6) -> ()  [unwired: 9 in, 2 out]
          }
        }
      }
      event "Log Button": Mouse Enter {
        n609 = event-data() -> ()  [unwired: 1 in, 4 out]
        n610 = property on="Log Button" class="Bool (strict)"() -> ("DisabledEnum"=w770:T9)  [unwired: 2 in, 2 out]
        n611 = Equal?(x=w770, y=T9."Enabled" ("Disabled")) -> (x = y?=w771:bool)
        n612 = case shown="True" w771 {
          frame False {
          }
          frame True {
            n613 = property on="Log Button" class="Bool (strict)"("BoolText.TextColor"=u32 16448250) -> ()  [unwired: 2 in, 2 out]
            n614 = property on="Log Button" class="Bool (strict)"("Colors [4]"=cluster{u32, u32}[] [{16777216, 6254465}]) -> ()  [unwired: 2 in, 2 out]
            n615 = call-poly <vilib>:"Set Cursor.vi"("icon"=u16 6) -> ()  [unwired: 9 in, 2 out]
          }
        }
      }
      event "Save Log": Mouse Enter {
        n616 = event-data() -> ()  [unwired: 1 in, 4 out]
        n617 = property on="Save Log" class="Bool (strict)"() -> ("DisabledEnum"=w776:T9)  [unwired: 2 in, 2 out]
        n618 = Equal?(x=w776, y=T9."Enabled" ("Disabled")) -> (x = y?=w777:bool)
        n619 = case shown="True" w777 {
          frame False {
          }
          frame True {
            n620 = property on="Save Log" class="Bool (strict)"("BoolText.TextColor"=u32 16448250) -> ()  [unwired: 2 in, 2 out]
            n621 = property on="Save Log" class="Bool (strict)"("Colors [4]"=cluster{u32, u32}[] [{16777216, 6254465}]) -> ()  [unwired: 2 in, 2 out]
            n622 = call-poly <vilib>:"Set Cursor.vi"("icon"=u16 6) -> ()  [unwired: 9 in, 2 out]
          }
        }
      }
      event "Clear": Mouse Enter {
        n623 = event-data() -> ()  [unwired: 1 in, 4 out]
        n624 = property on="Clear" class="Bool (strict)"() -> ("DisabledEnum"=w782:T9)  [unwired: 2 in, 2 out]
        n625 = Equal?(x=w782, y=T9."Enabled" ("Disabled")) -> (x = y?=w783:bool)
        n626 = case shown="True" w783 {
          frame False {
          }
          frame True {
            n627 = property on="Clear" class="Bool (strict)"("BoolText.TextColor"=u32 16448250) -> ()  [unwired: 2 in, 2 out]
            n628 = property on="Clear" class="Bool (strict)"("Colors [4]"=cluster{u32, u32}[] [{16777216, 6254465}]) -> ()  [unwired: 2 in, 2 out]
            n629 = call-poly <vilib>:"Set Cursor.vi"("icon"=u16 6) -> ()  [unwired: 9 in, 2 out]
          }
        }
      }
      event "Export": Mouse Enter {
        n630 = event-data() -> ()  [unwired: 1 in, 4 out]
        n631 = property on="Export" class="Bool (strict)"() -> ("DisabledEnum"=w788:T9)  [unwired: 2 in, 2 out]
        n632 = Equal?(x=w788, y=T9."Enabled" ("Disabled")) -> (x = y?=w789:bool)
        n633 = case shown="True" w789 {
          frame False {
          }
          frame True {
            n634 = property on="Export" class="Bool (strict)"("BoolText.TextColor"=u32 16448250) -> ()  [unwired: 2 in, 2 out]
            n635 = property on="Export" class="Bool (strict)"("Colors [4]"=cluster{u32, u32}[] [{16777216, 6254465}]) -> ()  [unwired: 2 in, 2 out]
            n636 = call-poly <vilib>:"Set Cursor.vi"("icon"=u16 6) -> ()  [unwired: 9 in, 2 out]
          }
        }
      }
      event "help": Mouse Enter {
        n637 = event-data() -> ()  [unwired: 1 in, 4 out]
        n638 = property on="help" class="Bool (strict)"() -> ("DisabledEnum"=w794:T9)  [unwired: 2 in, 2 out]
        n639 = Equal?(x=w794, y=T9."Enabled" ("Disabled")) -> (x = y?=w795:bool)
        n640 = case shown="True" w795 {
          frame False {
          }
          frame True {
            n641 = property on="help" class="Bool (strict)"("BoolText.TextColor"=u32 16448250) -> ()  [unwired: 2 in, 2 out]
            n642 = property on="help" class="Bool (strict)"("Colors [4]"=cluster{u32, u32}[] [{16777216, 6254465}]) -> ()  [unwired: 2 in, 2 out]
            n643 = call-poly <vilib>:"Set Cursor.vi"("icon"=u16 6) -> ()  [unwired: 9 in, 2 out]
          }
        }
      }
      event "Home": Mouse Enter {
        n644 = event-data() -> ()  [unwired: 1 in, 4 out]
        n645 = property on="Home" class="Bool (strict)"() -> ("DisabledEnum"=w800:T9)  [unwired: 2 in, 2 out]
        n646 = Equal?(x=w800, y=T9."Enabled" ("Disabled")) -> (x = y?=w801:bool)
        n647 = case shown="True" w801 {
          frame False {
          }
          frame True {
            n648 = property on="Home" class="Bool (strict)"("BoolText.TextColor"=u32 16448250) -> ()  [unwired: 2 in, 2 out]
            n649 = property on="Home" class="Bool (strict)"("Colors [4]"=cluster{u32, u32}[] [{16777216, 6254465}]) -> ()  [unwired: 2 in, 2 out]
            n650 = call-poly <vilib>:"Set Cursor.vi"("icon"=u16 6) -> ()  [unwired: 9 in, 2 out]
          }
        }
      }
      event "A / M": Mouse Enter {
        n651 = event-data() -> ()  [unwired: 1 in, 4 out]
        n652 = call-poly <vilib>:"Set Cursor.vi"("icon"=u16 6) -> ()  [unwired: 9 in, 2 out]
      }
      event "Add Load": Mouse Enter {
        n653 = event-data() -> ()  [unwired: 1 in, 4 out]
        n654 = call-poly <vilib>:"Set Cursor.vi"("icon"=u16 6) -> ()  [unwired: 9 in, 2 out]
      }
      event "Radio Buttons.On / Off Control": Mouse Enter {
        n655 = event-data() -> ()  [unwired: 1 in, 4 out]
        n656 = call-poly <vilib>:"Set Cursor.vi"("icon"=u16 6) -> ()  [unwired: 9 in, 2 out]
      }
      event "Radio Buttons.On / Off Control": Mouse Leave {
        n657 = event-data() -> ()  [unwired: 1 in, 4 out]
        n658 = call-poly <vilib>:"Set Cursor.vi"("icon"=u16 1) -> ()  [unwired: 9 in, 2 out]
      }
      event "Radio Buttons.P Mode": Mouse Enter {
        n659 = event-data() -> ()  [unwired: 1 in, 4 out]
        n660 = call-poly <vilib>:"Set Cursor.vi"("icon"=u16 6) -> ()  [unwired: 9 in, 2 out]
      }
      event "Radio Buttons.P Mode": Mouse Leave {
        n661 = event-data() -> ()  [unwired: 1 in, 4 out]
        n662 = call-poly <vilib>:"Set Cursor.vi"("icon"=u16 1) -> ()  [unwired: 9 in, 2 out]
      }
      event "Run": Mouse Leave {
        n663 = event-data() -> ()  [unwired: 1 in, 4 out]
        n664 = property on="Run" class="Bool (strict)"() -> ("DisabledEnum"=w813:T9)  [unwired: 2 in, 2 out]
        n665 = Equal?(x=w813, y=T9."Disabled" ("Disabled")) -> (x = y?=w811:bool)
        n666 = case shown="False" w811 {
          frame False {
            n667 = property on="Run" class="Bool (strict)"("BoolText.TextColor"=u32 9868950) -> ()  [unwired: 2 in, 2 out]
            n668 = property on="Run" class="Bool (strict)"("Colors [4]"=cluster{u32, u32}[] [{16777216, 16777215}]) -> ()  [unwired: 2 in, 2 out]
            n669 = call-poly <vilib>:"Set Cursor.vi"("icon"=u16 1) -> ()  [unwired: 9 in, 2 out]
          }
          frame True {
          }
        }
      }
      event "Pause": Mouse Leave {
        n670 = event-data() -> ()  [unwired: 1 in, 4 out]
        n671 = flat-sequence {
          frame #0 {
            n672 = property on="Pause" class="Bool (strict)"() -> ("DisabledEnum"=w818:T9)  [unwired: 2 in, 2 out]
            n673 = Equal?(x=w818, y=T9."Enabled" ("Disabled")) -> (x = y?=w819:bool)
            n674 = case shown="True" w819 {
              frame False {
              }
              frame True {
                n675 = property on="Pause" class="Bool (strict)"("BoolText.TextColor"=u32 9868950) -> ()  [unwired: 2 in, 2 out]
                n676 = property on="Pause" class="Bool (strict)"("Colors [4]"=cluster{u32, u32}[] [{16777216, 16777215}]) -> ()  [unwired: 2 in, 2 out]
                n677 = call-poly <vilib>:"Set Cursor.vi"("icon"=u16 1) -> ()  [unwired: 9 in, 2 out]
              }
            }
          }
          frame #1 {
            n678 = local read "Pause"() -> (w823:bool)
            n679 = case shown="True" w823 {
              frame False {
              }
              frame True {
                n680 = property on="Pause" class="Bool (strict)"("Colors [4]"=cluster{u32, u32}[] [{16777216, 32768}]) -> ()  [unwired: 2 in, 2 out]
              }
            }
          }
        }
      }
      event "Single Step": Mouse Leave {
        n681 = event-data() -> ()  [unwired: 1 in, 4 out]
        n682 = property on="Single Step" class="Bool (strict)"() -> ("DisabledEnum"=w827:T9)  [unwired: 2 in, 2 out]
        n683 = Equal?(x=w827, y=T9."Enabled" ("Disabled")) -> (x = y?=w825:bool)
        n684 = case shown="True" w825 {
          frame False {
          }
          frame True {
            n685 = property on="Single Step" class="Bool (strict)"("BoolText.TextColor"=u32 9868950) -> ()  [unwired: 2 in, 2 out]
            n686 = property on="Single Step" class="Bool (strict)"("Colors [4]"=cluster{u32, u32}[] [{16777216, 16777215}]) -> ()  [unwired: 2 in, 2 out]
            n687 = call-poly <vilib>:"Set Cursor.vi"("icon"=u16 1) -> ()  [unwired: 9 in, 2 out]
          }
        }
      }
      event "Stop": Mouse Leave {
        n688 = event-data() -> ()  [unwired: 1 in, 4 out]
        n689 = property on="Stop" class="Bool (strict)"() -> ("DisabledEnum"=w833:T9)  [unwired: 2 in, 2 out]
        n690 = Equal?(x=w833, y=T9."Enabled" ("Disabled")) -> (x = y?=w831:bool)
        n691 = case shown="True" w831 {
          frame False {
          }
          frame True {
            n692 = property on="Stop" class="Bool (strict)"("BoolText.TextColor"=u32 9868950) -> ()  [unwired: 2 in, 2 out]
            n693 = property on="Stop" class="Bool (strict)"("Colors [4]"=cluster{u32, u32}[] [{16777216, 16777215}]) -> ()  [unwired: 2 in, 2 out]
            n694 = call-poly <vilib>:"Set Cursor.vi"("icon"=u16 1) -> ()  [unwired: 9 in, 2 out]
          }
        }
      }
      event "Log Button": Mouse Leave {
        n695 = event-data() -> ()  [unwired: 1 in, 4 out]
        n696 = flat-sequence {
          frame #0 {
            n697 = property on="Log Button" class="Bool (strict)"() -> ("DisabledEnum"=w839:T9)  [unwired: 2 in, 2 out]
            n698 = Equal?(x=w839, y=T9."Enabled" ("Disabled")) -> (x = y?=w837:bool)
            n699 = case shown="True" w837 {
              frame False {
              }
              frame True {
                n700 = property on="Log Button" class="Bool (strict)"("BoolText.TextColor"=u32 9868950) -> ()  [unwired: 2 in, 2 out]
                n701 = property on="Log Button" class="Bool (strict)"("Colors [4]"=cluster{u32, u32}[] [{16777216, 16777215}]) -> ()  [unwired: 2 in, 2 out]
                n702 = call-poly <vilib>:"Set Cursor.vi"("icon"=u16 1) -> ()  [unwired: 9 in, 2 out]
              }
            }
          }
          frame #1 {
            n703 = local read "Log Button"() -> (w843:bool)
            n704 = case shown="True" w843 {
              frame False {
              }
              frame True {
                n705 = property on="Log Button" class="Bool (strict)"("Colors [4]"=cluster{u32, u32}[] [{16777216, 32768}]) -> ()  [unwired: 2 in, 2 out]
              }
            }
          }
        }
      }
      event "Save Log": Mouse Leave {
        n706 = event-data() -> ()  [unwired: 1 in, 4 out]
        n707 = property on="Save Log" class="Bool (strict)"() -> ("DisabledEnum"=w847:T9)  [unwired: 2 in, 2 out]
        n708 = Equal?(x=w847, y=T9."Enabled" ("Disabled")) -> (x = y?=w845:bool)
        n709 = case shown="True" w845 {
          frame False {
          }
          frame True {
            n710 = property on="Save Log" class="Bool (strict)"("BoolText.TextColor"=u32 9868950) -> ()  [unwired: 2 in, 2 out]
            n711 = property on="Save Log" class="Bool (strict)"("Colors [4]"=cluster{u32, u32}[] [{16777216, 16777215}]) -> ()  [unwired: 2 in, 2 out]
            n712 = call-poly <vilib>:"Set Cursor.vi"("icon"=u16 1) -> ()  [unwired: 9 in, 2 out]
          }
        }
      }
      event "Clear": Mouse Leave {
        n713 = event-data() -> ()  [unwired: 1 in, 4 out]
        n714 = property on="Clear" class="Bool (strict)"() -> ("DisabledEnum"=w853:T9)  [unwired: 2 in, 2 out]
        n715 = Equal?(x=w853, y=T9."Enabled" ("Disabled")) -> (x = y?=w851:bool)
        n716 = case shown="True" w851 {
          frame False {
          }
          frame True {
            n717 = property on="Clear" class="Bool (strict)"("BoolText.TextColor"=u32 9868950) -> ()  [unwired: 2 in, 2 out]
            n718 = property on="Clear" class="Bool (strict)"("Colors [4]"=cluster{u32, u32}[] [{16777216, 16777215}]) -> ()  [unwired: 2 in, 2 out]
            n719 = call-poly <vilib>:"Set Cursor.vi"("icon"=u16 1) -> ()  [unwired: 9 in, 2 out]
          }
        }
      }
      event "Export": Mouse Leave {
        n720 = event-data() -> ()  [unwired: 1 in, 4 out]
        n721 = property on="Export" class="Bool (strict)"() -> ("DisabledEnum"=w859:T9)  [unwired: 2 in, 2 out]
        n722 = Equal?(x=w859, y=T9."Enabled" ("Disabled")) -> (x = y?=w857:bool)
        n723 = case shown="True" w857 {
          frame False {
          }
          frame True {
            n724 = property on="Export" class="Bool (strict)"("BoolText.TextColor"=u32 9868950) -> ()  [unwired: 2 in, 2 out]
            n725 = property on="Export" class="Bool (strict)"("Colors [4]"=cluster{u32, u32}[] [{16777216, 16777215}]) -> ()  [unwired: 2 in, 2 out]
            n726 = call-poly <vilib>:"Set Cursor.vi"("icon"=u16 1) -> ()  [unwired: 9 in, 2 out]
          }
        }
      }
      event "help": Mouse Leave {
        n727 = event-data() -> ()  [unwired: 1 in, 4 out]
        n728 = property on="help" class="Bool (strict)"("BoolText.TextColor"=u32 9868950) -> ()  [unwired: 2 in, 2 out]
        n729 = property on="help" class="Bool (strict)"("Colors [4]"=cluster{u32, u32}[] [{16777216, 16777215}]) -> ()  [unwired: 2 in, 2 out]
        n730 = call-poly <vilib>:"Set Cursor.vi"("icon"=u16 1) -> ()  [unwired: 9 in, 2 out]
      }
      event "Home": Mouse Leave {
        n731 = event-data() -> ()  [unwired: 1 in, 4 out]
        n732 = property on="Home" class="Bool (strict)"() -> ("DisabledEnum"=w868:T9)  [unwired: 2 in, 2 out]
        n733 = Equal?(x=w868, y=T9."Enabled" ("Disabled")) -> (x = y?=w866:bool)
        n734 = case shown="True" w866 {
          frame False {
          }
          frame True {
            n735 = property on="Home" class="Bool (strict)"("BoolText.TextColor"=u32 9868950) -> ()  [unwired: 2 in, 2 out]
            n736 = property on="Home" class="Bool (strict)"("Colors [4]"=cluster{u32, u32}[] [{16777216, 16777215}]) -> ()  [unwired: 2 in, 2 out]
            n737 = call-poly <vilib>:"Set Cursor.vi"("icon"=u16 1) -> ()  [unwired: 9 in, 2 out]
          }
        }
      }
      event "A / M": Mouse Leave {
        n738 = event-data() -> ()  [unwired: 1 in, 4 out]
        n739 = call-poly <vilib>:"Set Cursor.vi"("icon"=u16 1) -> ()  [unwired: 9 in, 2 out]
      }
      event "Add Load": Mouse Leave {
        n740 = event-data() -> ()  [unwired: 1 in, 4 out]
        n741 = call-poly <vilib>:"Set Cursor.vi"("icon"=u16 1) -> ()  [unwired: 9 in, 2 out]
      }
      event "Run": Value Change {
        n742 = event-data() -> ()  [unwired: 1 in, 6 out]
        n743 = local read "Run"() -> (w874:bool)
        n744 = case shown="True" w874 {
          frame False {
          }
          frame True {
            n745 = property on="Run" class="Bool (strict)"("BoolText.TextColor"=u32 9868950) -> ()  [unwired: 2 in, 2 out]
            n746 = property on="Run" class="Bool (strict)"("Colors [4]"=cluster{u32, u32}[] [{16777216, 32768}]) -> ()  [unwired: 2 in, 2 out]
          }
        }
      }
      event "Pause": Value Change {
        n747 = event-data() -> ()  [unwired: 1 in, 6 out]
      }
      event "Single Step": Value Change {
        n748 = event-data() -> ()  [unwired: 1 in, 6 out]
        n749 = flat-sequence {
          frame #0 {
            n750 = local read "Single Step"() -> (w878:bool)
            n751 = case shown="True" w878 {
              frame False {
              }
              frame True {
                n752 = property on="Single Step" class="Bool (strict)"("BoolText.TextColor"=u32 9868950) -> ()  [unwired: 2 in, 2 out]
                n753 = property on="Single Step" class="Bool (strict)"("Colors [4]"=cluster{u32, u32}[] [{16777216, 32768}]) -> ()  [unwired: 2 in, 2 out]
              }
            }
            n754 = Wait Until Next ms Multiple(millisecond multiple=u32 200) -> ()  [unwired: 1 out]
          }
          frame #1 {
            n755 = property on="Single Step" class="Bool (strict)"("Colors [4]"=cluster{u32, u32}[] [{16777216, 16777215}]) -> ()  [unwired: 2 in, 2 out]
          }
        }
      }
      event "Stop": Value Change {
        n756 = event-data() -> ()  [unwired: 1 in, 6 out]
        n757 = property on="Stop" class="Bool (strict)"("BoolText.TextColor"=u32 9868950) -> ()  [unwired: 2 in, 2 out]
        n758 = property on="Stop" class="Bool (strict)"("Colors [4]"=cluster{u32, u32}[] [{16777216, 32768}]) -> ()  [unwired: 2 in, 2 out]
        n759 = call "Stop"() -> ("OK"=w883:bool)  [unwired: 10 in, 1 out]
        n760 = local write "Stop Flag"(w883) -> ()
        n761 = Wait For Front Panel Activity(3:TRUE ("do not wait! (False)")) -> ()  [unwired: 2 in, 1 out]
      }
      event "Log Button": Value Change {
        n762 = event-data() -> ()  [unwired: 1 in, 6 out]
        n763 = local read "Log Button"() -> (w886:bool)
        n764 = case shown="False" w886 {
          frame False {
            n765 = local write "Tab Control 2"(T4."Controller Parameters" ("Tab Control 2")) -> ()
            n766 = property on="Log" class="Bool (strict)"("Blinking"=FALSE) -> ()  [unwired: 2 in, 2 out]
          }
          frame True {
            n767 = property on="Log Button" class="Bool (strict)"("BoolText.TextColor"=u32 9868950) -> ()  [unwired: 2 in, 2 out]
            n768 = property on="Log Button" class="Bool (strict)"("Colors [4]"=cluster{u32, u32}[] [{16777216, 32768}]) -> ()  [unwired: 2 in, 2 out]
            n769 = local write "Tab Control 2"(T4."Log Table" ("Tab Control 2")) -> ()
            n770 = property on="Log" class="Bool (strict)"("Blinking"=TRUE) -> ()  [unwired: 2 in, 2 out]
          }
        }
      }
      event "Save Log": Value Change {
        n771 = event-data() -> ()  [unwired: 1 in, 6 out]
        n772 = local write "Save Log"(FALSE ("Save Log")) -> ()
        n773 = property on="Save Log" class="Bool (strict)"("BoolText.TextColor"=u32 9868950) -> ()  [unwired: 2 in, 2 out]
        n774 = property on="Save Log" class="Bool (strict)"("Colors [4]"=cluster{u32, u32}[] [{16777216, 32768}]) -> ()  [unwired: 2 in, 2 out]
        n775 = invoke on="Table" class="Tbl (strict)" method="Export Data to Excel"() -> ()  [unwired: 3 in, 3 out]
      }
      event "Clear": Value Change {
        n776 = event-data() -> ()  [unwired: 1 in, 6 out]
        n777 = property on="Clear" class="Bool (strict)"("BoolText.TextColor"=u32 9868950) -> ()  [unwired: 2 in, 2 out]
        n778 = property on="Clear" class="Bool (strict)"("Colors [4]"=cluster{u32, u32}[] [{16777216, 32768}]) -> ()  [unwired: 2 in, 2 out]
        n779 = Two Button Dialog(message="Data will be cleared.\nDo you want to proceed?") -> (T button?=w897:bool)  [unwired: 2 in]
        n780 = case shown="False" w897 {
          frame False {
            n781 = local write "Clear"(FALSE ("Clear Button")) -> ()
          }
          frame True {
            n782 = invoke on="Table" class="Tbl (strict)" method="Reinit To Default"() -> ()  [unwired: 3 in, 3 out]
            n783 = local write "Log Count"(0.0 ("Log Count")) -> ()
            n784 = local write "Clear"(FALSE ("Clear Button")) -> ()
          }
        }
      }
      event "Export": Value Change {
        n785 = event-data() -> ()  [unwired: 1 in, 6 out]
        n786 = local write "Export"(FALSE ("Export")) -> ()
        n787 = property on="Export" class="Bool (strict)"("BoolText.TextColor"=u32 9868950) -> ()  [unwired: 2 in, 2 out]
        n788 = property on="Export" class="Bool (strict)"("Colors [4]"=cluster{u32, u32}[] [{16777216, 32768}]) -> ()  [unwired: 2 in, 2 out]
        n789 = invoke on="Waveform Chart" class="WFChart (strict)" method="Get Image"() -> ("image data"=w904:T13)  [unwired: 6 in, 5 out]
        n790 = call <vilib>:"Write JPEG File.vi"("image data"=w904) -> ("error out"=w903:errorcluster)  [unwired: 9 in, 1 out]
      }
      event "Home": Value Change {
        n791 = event-data() -> ()  [unwired: 1 in, 6 out]
        n792 = local read "Home"() -> (w908:bool)
      }
      event "help": Value Change {
        n793 = event-data() -> ()  [unwired: 1 in, 1 out]
        n794 = call-poly <vilib>:"Set Cursor.vi"("icon"=u16 1) -> ()  [unwired: 9 in, 2 out]
        n795 = call <vilib>:"Application Directory.vi"() -> ("Application Directory"=w927:path)
        n796 = call <vilib>:"Open Registry Key.vi"("security access mask (KEY_READ | KEY_WRITE)"=Registry_SAM."KEY_READ", "subkey"="Software\\Adobe\\Acrobat\\Exe", "root key (HKEY_LOCAL_MACHINE)"=Registry_RtKey."HKEY_CLASSES_ROOT") -> ("error out"=w915:errorcluster, "refnum out"=w914:T14)  [unwired: 7 in]
        n797 = Path To String(path=w927) -> (string=w925:string)
        n798 = call-poly <vilib>:"Read Registry Value Simple.vi"("error in (no error)"=w915, "value"="", "refnum"=w914) -> ("error out"=w918:errorcluster, "String/Binary data"=w923:string, "refnum out"=w919:T14)  [unwired: 3 in, 1 out]
        n799 = Concatenate Strings(w925, "\\User Guide\\ACE400.pdf" ("string")) -> (w928:string)
        n800 = local write "help"(FALSE ("Help Button")) -> ()
        n801 = Format Into String(format string=" \"%s\"", initial string=w923, w928) -> (resulting string=w922:string)  [unwired: 1 in, 1 out]
        n802 = call <vilib>:"Close Registry Key.vi"("error in (no error)"=w918, "refnum"=w919) -> ("error out"=w910:errorcluster)  [unwired: 5 in]
        n803 = call <vilib>:"System Exec.vi"("wait until completion? (T)"=FALSE, "command line"=w922) -> ("error out"=w912:errorcluster)  [unwired: 6 in, 3 out]
        n804 = case shown="Error" w912 {
          frame No Error {
          }
          frame Error {
            n805 = call "Display Message to User"() -> ()  [unwired: 10 in, 2 out]
            n806 = property on="help" class="Bool (strict)"("Colors [4]"=cluster{u32, u32}[] [{16777216, 16777215}]) -> ()  [unwired: 2 in, 2 out]
          }
        }
      }
    }
  }
